vi "ActiveObjects_DynamicEvents.vi"(7 "Action":T2=enum."GeneratePattern", 8 "error in (no error)":errorcluster, 10 "DataIn":variant, 11 "ClassRefToActOn":refnum<vi>) -> (0 "error out":errorcluster, 1 "Name":string, 2 "DataOut":variant, 3 "Cancelled":bool)   [LabVIEW 2020]
uses:
  Provider_BaseClassInterface/BaseProvider_SubVIs/BaseProvider_DesignPatternsActions.ctl
  Common/LvClass_class/GDSLvClass_ProviderTypes.ctl
  Provider_EndevoGOOP400/EndevoG4ProviderName.ctl
  Common/CommonVIs/CommonVIs_AttributeDataType.ctl
  <vilib>/picture/picture.llb/imagedata.ctl
  Common/LvIcon_class/subvis/GDSLvIcon_TextDataType.ctl
  Common/LvIcon_class/GDSLvIcon_WordCompressionType.ctl
  Common/LvIcon_class/GDSLvIcon_TextAlignment.ctl
  <vilib>/Utility/lvfile.llb/NI_FileType.lvlib
panel:
  out "NameExist4":string
  in  "AddWindowControlVI":bool
  in  "WindowControlName":string caption="Enter process window control VI name"
  in  "ProcessCreation":T1(ring) caption="Process creation"
  out "NameExist1":string
  out "NameExist3":string
  out "NameExist2":string
  in  "AddInDestructor":bool
  in  "AddInConstructor":bool
  in  "StopName":string caption="Enter Stop Process Name"
  in  "StartName":string caption="Enter Start Process Name"
  in  "_Cancel":bool
  in  "_OK":bool
  in  "ProcessName":string caption="Enter Active Process Name"
  # "Active Object using Dymanic Events"
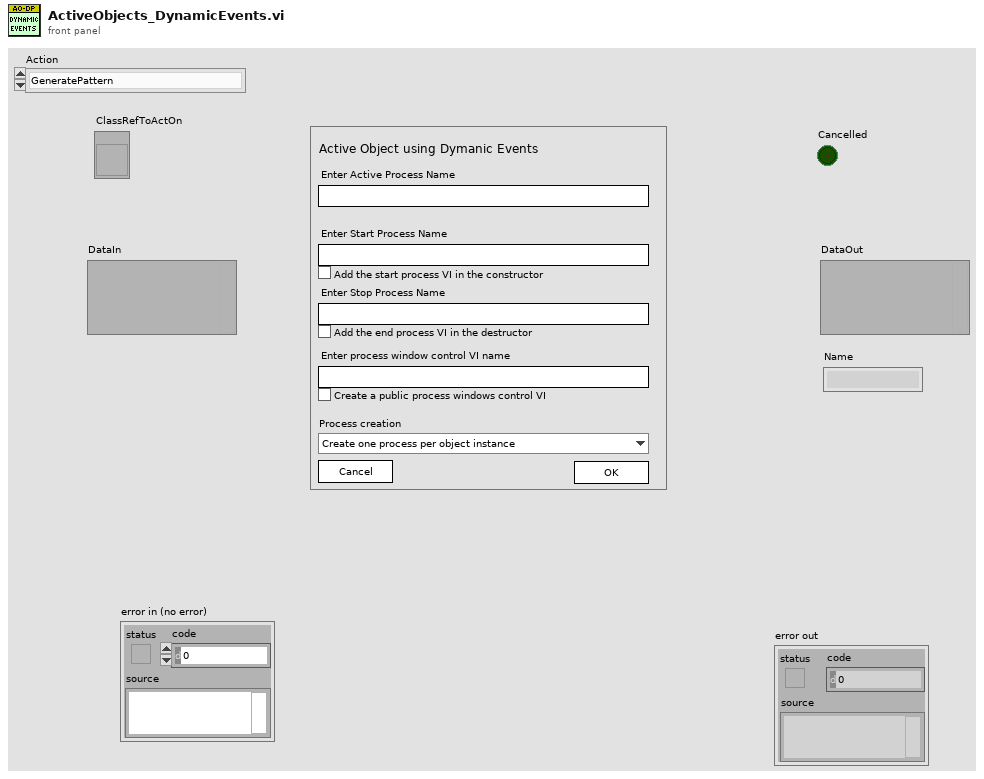
[diagram p1: front panel]
types:
  T1 = enum16{"Create one process per object instance", "Create only one process for this class"}
  T2 = typedef "BaseProvider_DesignPatternsActions.ctl" = enum16{"AddPatternDialog", "GeneratePattern", "RemovePattern", "CreatePatternMethod", "UpdatePattern"}
  T3 = typedef "GDSLvClass_ProviderTypes.ctl" = enum16{"UnKnown(LabVOOP)", "Native", "EndevoGOOP3", "OpenG(RootObject)", "OpenG(OpenG_Object)", "EndevoGOOP4", "JKI1"}
  T4 = cluster{"Data":cluster{"ProcessName":string, "StartName":string, "StopName":string, "AddInConstructor":bool, "AddInDestructor":bool, "ProcessCreation":enum16{"Create one process per object instance", "Create only one process for this class"}, "WindowControlName":string, "AddWindowControlVI":bool}, "ClassFolder":path, "SupportFolder":path, "ProcessCtl":refnum<vi>, "ProtectedFolder":refnum<vi>, "ProcessVI":refnum<vi>, "StartVI":refnum<vi>, "StopVI":refnum<vi>, "Application":refnum<vi>, "RepositoryVI":refnum<vi>, "ProcessIdRef":refnum<vi>, "ProcessRepository":path, "ClassProvider":T3, "TemplateName":string, "VI_ToFind":path, "MethodTemplate":path, "VI":refnum<vi>, "VI_ToFindSingleton":path, "Name":string, "WindowControlVI":refnum<vi>, "ClassType":enum16{"4x4x4", "5x6x5", "6x8x6", "4x4x4_Singleton", "5x6x5_Singleton", "6x8x6_Singleton"}}
  T5 = cluster{"ProcessName":string, "StartName":string, "StopName":string, "AddInConstructor":bool, "AddInDestructor":bool, "ProcessCreation":enum16{"Create one process per object instance", "Create only one process for this class"}, "WindowControlName":string, "AddWindowControlVI":bool}
  T6 = enum8{"Enabled", "Disabled", "Disabled and Grayed Out"}
  T7 = cluster{"Cancelled":bool, "Files":path[], "ClassPath":path, "DataOut":variant, "Name":string}
  T8 = typedef "EndevoG4ProviderName.ctl" = enum16{"EndevoGOOP400"}
  T9 = enum16{"4x4x4", "5x6x5", "6x8x6", "4x4x4_Singleton", "5x6x5_Singleton", "6x8x6_Singleton"}
  T10 = enum32{"invalid VI type", "Standard VI", "Control VI", "Global VI", "Polymorphic VI", "Configuration VI", "SubSystem", "Facade VI", "Method VI"}
  T11 = typedef "GDSLvIcon_TextDataType.ctl" = cluster{"Text":string, "Allow Only Capital Chars":bool, "Compression":T12, "Alignment":T13}
  T12 = typedef "GDSLvIcon_WordCompressionType.ctl" = enum16{"Auto", "On", "Off"}
  T13 = typedef "GDSLvIcon_TextAlignment.ctl" = enum16{"Center", "Left", "Right"}
  T14 = typedef "imagedata.ctl" = cluster{"image type":i32, "image depth":i32, "image":u8[], "mask":u8[], "colors":u32[], "Rectangle":cluster{"left":i16, "top":i16, "right":i16, "bottom":i16}}
  T15 = typedef "GDSLvCLass_ClassSettingsType.ctl" = cluster{"ClassProviderName":string, "ClassTemplateUsed":string, "ClassTemplateVersion":string, "ClassDescription":string, "PlugIns":T16[], "ConnectorPanePattern":string}
  T16 = typedef "GDSLvClass_PlugIn.ctl" = cluster{"Type":T17, "ID":string, "Version":string, "Path":path, "Name":string, "Data":variant}
  T17 = typedef "GDSLvClass_PlugInTypes.ctl" = enum16{"DesignPattern", "MethodTypes"}
  T18 = typedef "GOOP400_Options.ctl" = cluster{"FlatFolderStructure":bool}
  T19 = enum32{"invalid scope", "public", "private", "protected"}[]
  T20 = typedef "CommonVIs_AttributeDataType.ctl" = enum16{"UINT8", "INT8", "UINT16", "INT16", "UINT32", "INT32", "UINT64", "INT64", "SGL", "DBL", "EXT", "CSG", "CDB", "CXT", "TimeStamp", "STRING", "PATH", "BOOL", "ENUM", "RefNum", "VIRefNum", "LabVIEW Class", "Cluster", "Variant", "TypeDef", "Waveform", "LabVIEW Object", "Other", "void", "Set", "Map"}
  T21 = typedef "GDSLvClass_IconSettingsType.ctl" = cluster{"Frame":u32, "Frame thickness":u8, "Header Background":u32, "Header Text":u32, "ColorPublic":u32, "ColorProtected":u32, "ColorPrivate":u32, "Body Text":u32, "ClassBodyIcon":string}
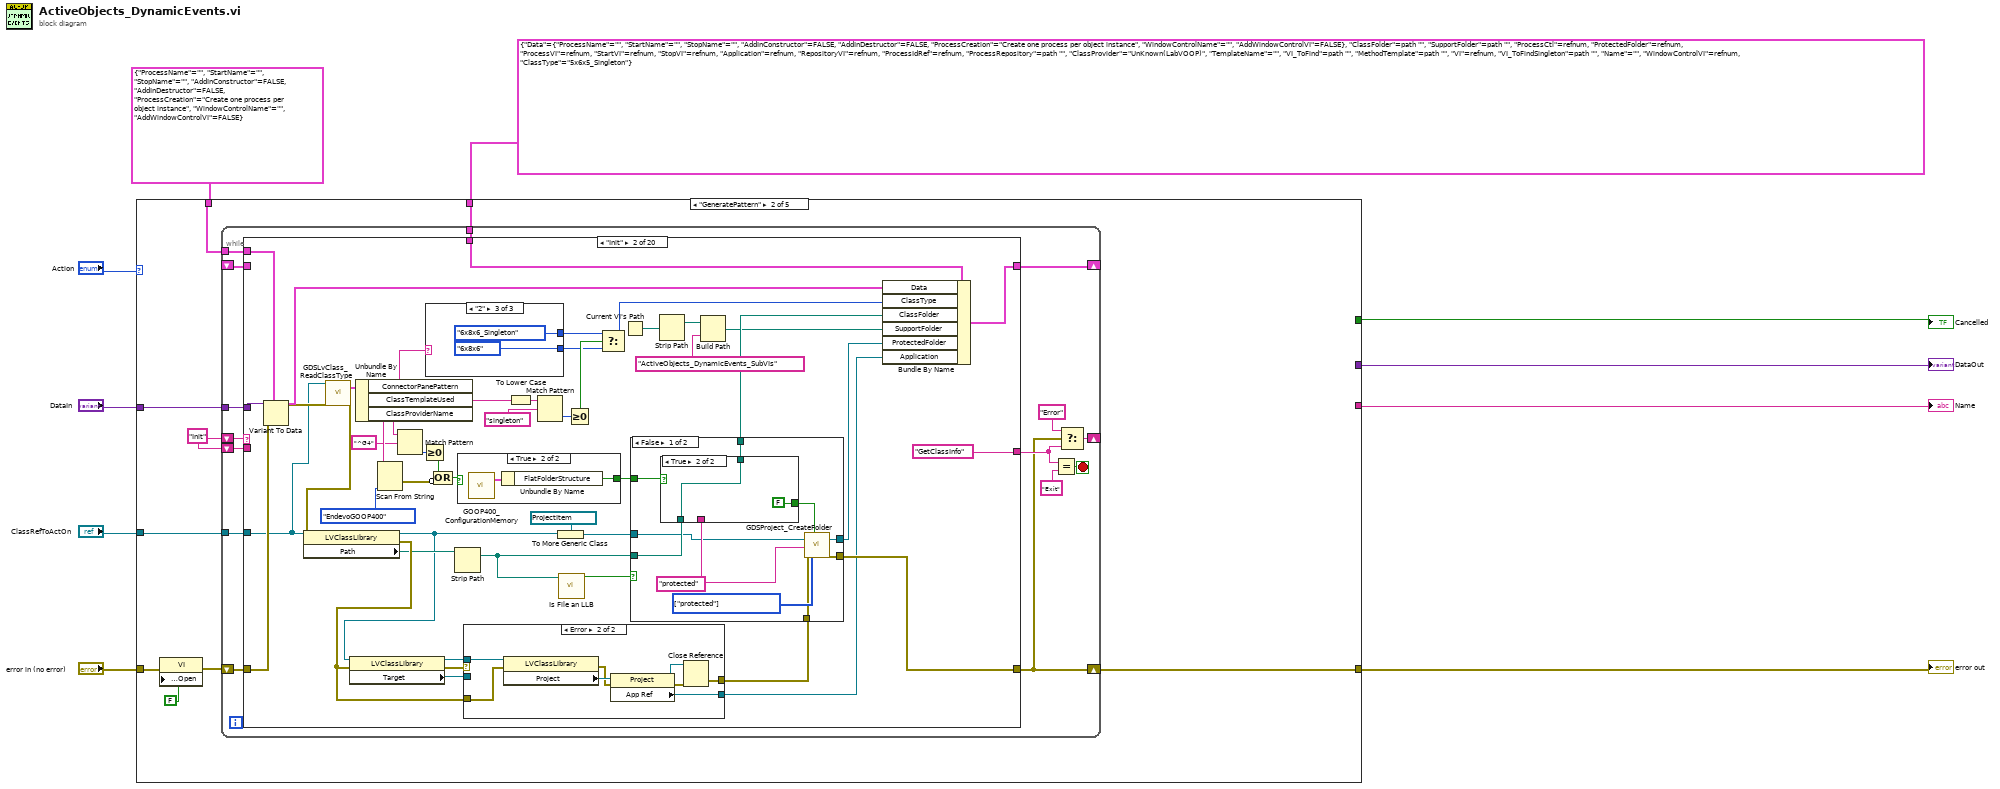
[diagram p0: block diagram]
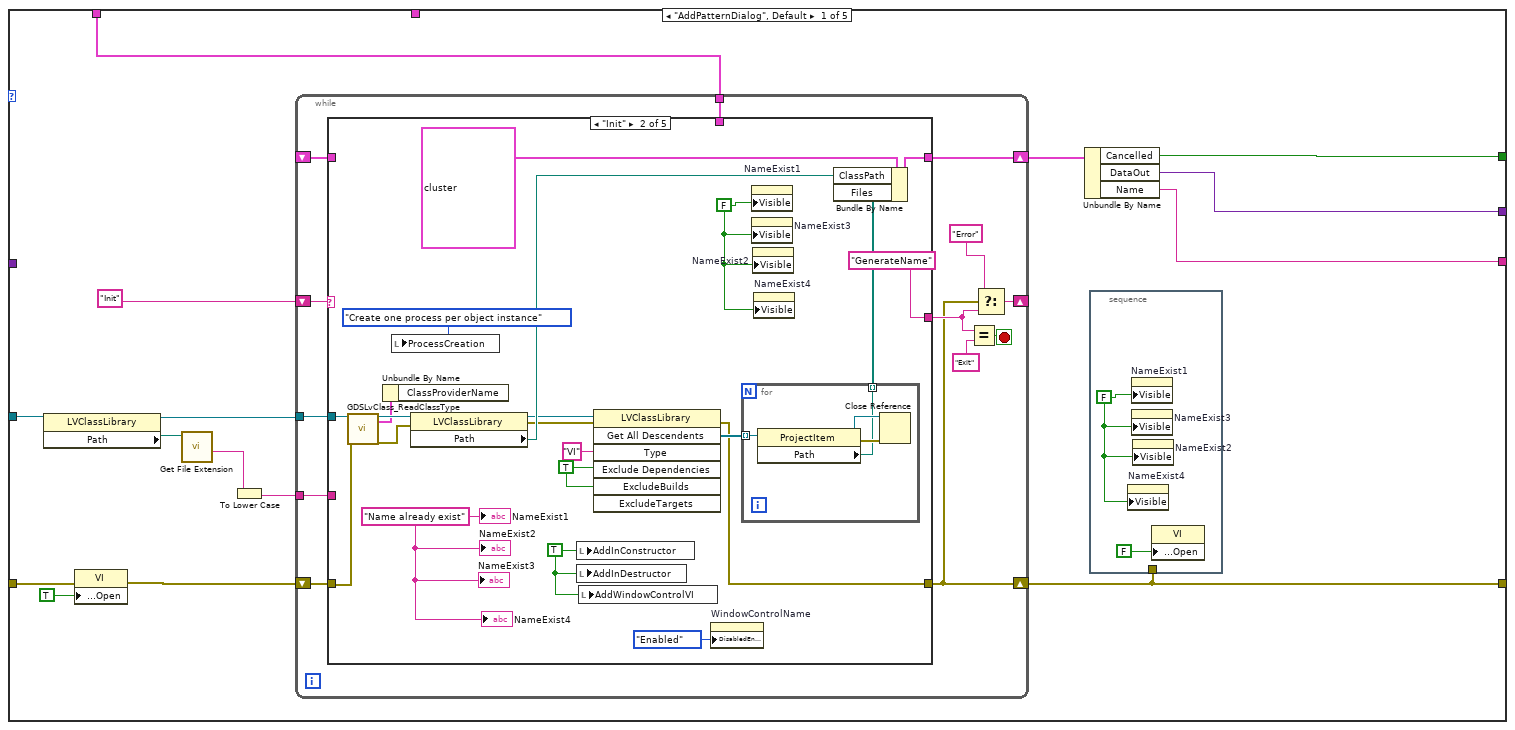
[diagram p2: hidden frame]
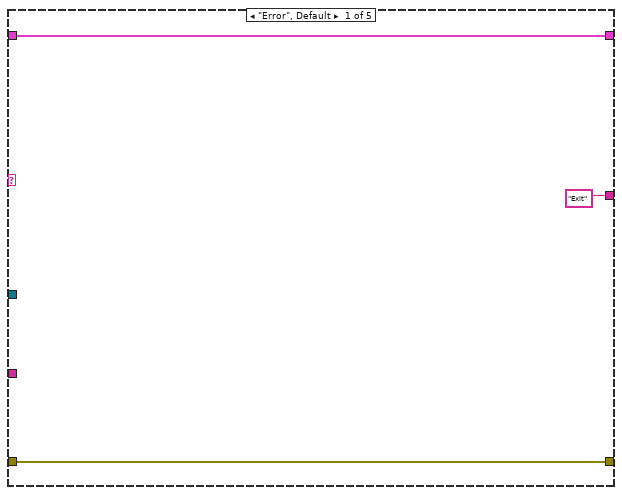
[diagram p3: hidden frame]
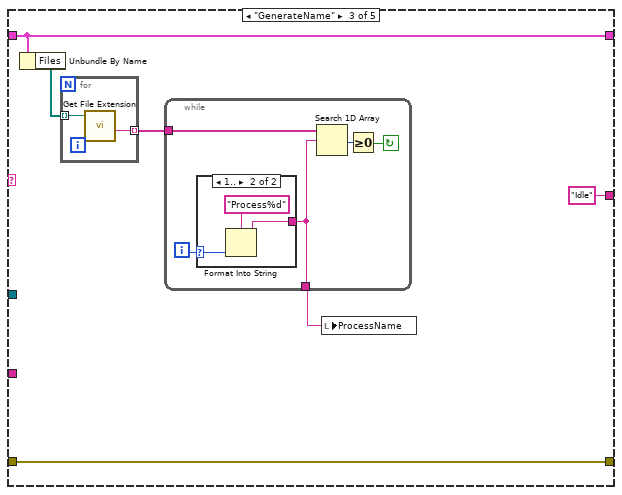
[diagram p4: hidden frame]
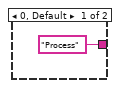
[diagram p5: hidden frame]
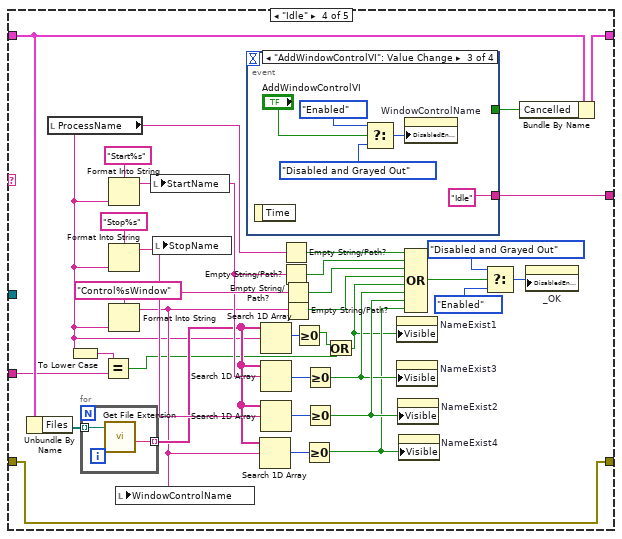
[diagram p6: hidden frame]
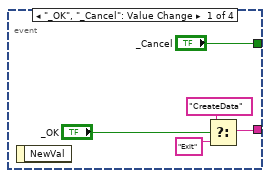
[diagram p7: hidden frame]
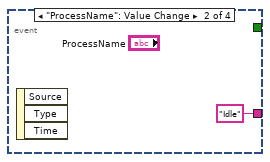
[diagram p8: hidden frame]
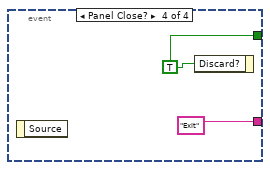
[diagram p9: hidden frame]
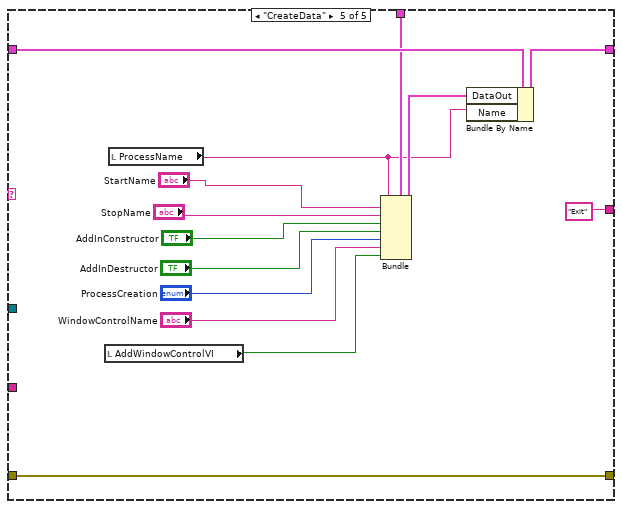
[diagram p10: hidden frame]
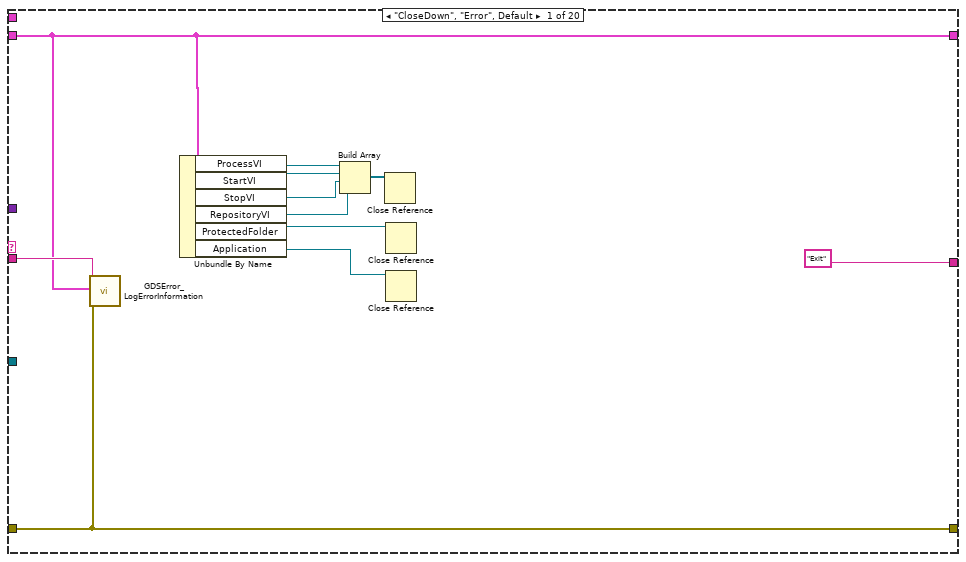
[diagram p11: hidden frame]
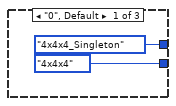
[diagram p13: hidden frame]
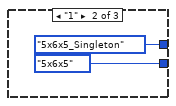
[diagram p14: hidden frame]
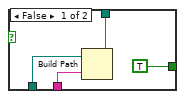
[diagram p15: hidden frame]
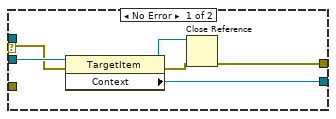
[diagram p17: hidden frame]
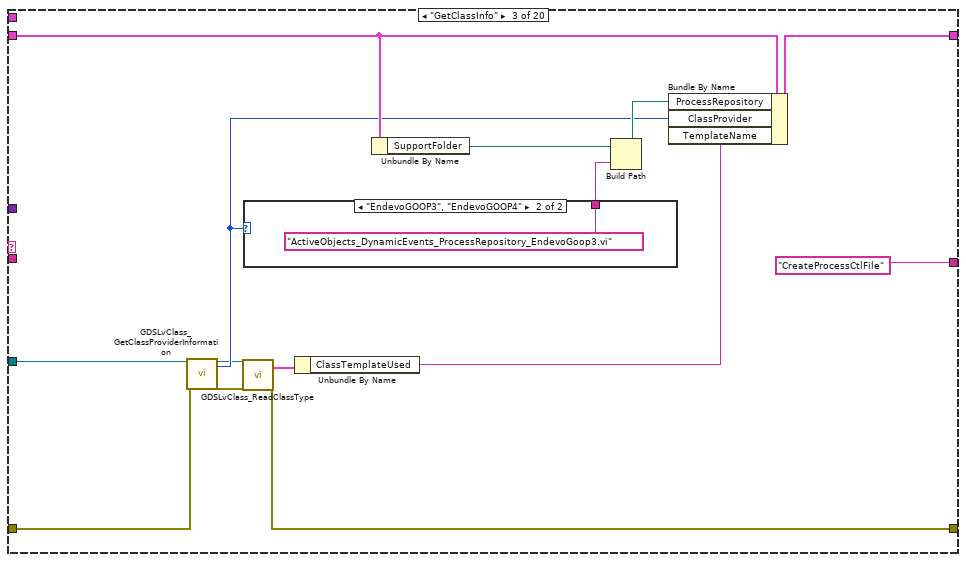
[diagram p18: hidden frame]
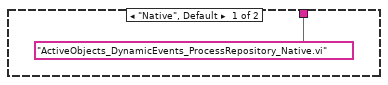
[diagram p19: hidden frame]
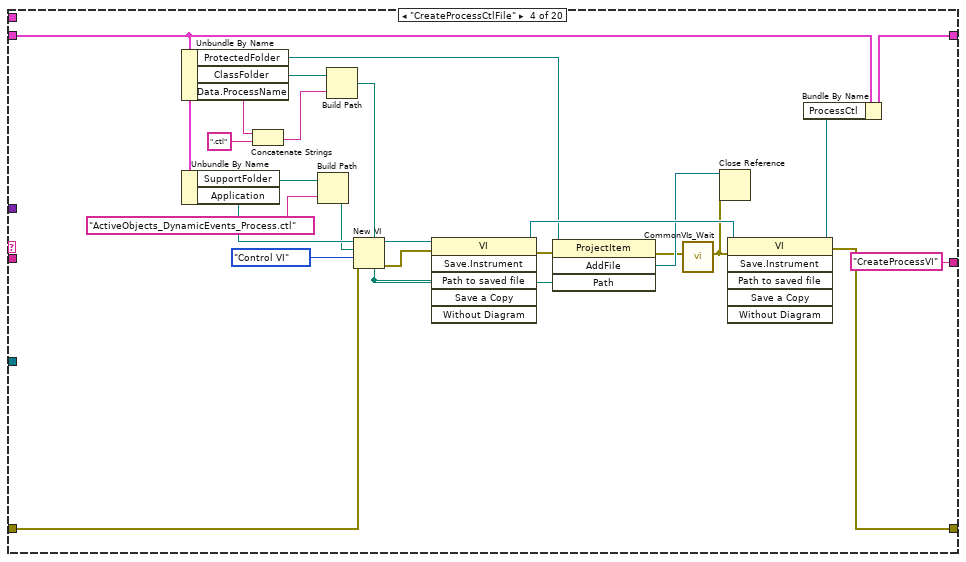
[diagram p20: hidden frame]
diagram:
  n1 = case shown="\"GeneratePattern\"" "Action" {
    tunnel: "error in (no error)" -> [w24 w151 w883 w884 w890]
    tunnel: [w21 w157 w883 w884 w885] -> w8
    tunnel: "ClassRefToActOn" -> [w15 w153 _ _ w889]
    tunnel: [w19 _ _ _ _] -> w6
    tunnel: [w18 _ _ _ _] -> w5
    tunnel: T5 {"ProcessName"="", "StartName"="", "StopName"="", "AddInConstructor"=FALSE, "AddInDestructor"=FALSE, "ProcessCreation"=enum."Create one process per object instance", "WindowControlName"="", "AddWindowControlVI"=FALSE} ("output cluster") -> [w17 w155 _ _ w886]
    tunnel: "DataIn" -> [_ w156 _ _ w888]
    tunnel: T4 {"Data"={"ProcessName"="", "StartName"="", "StopName"="", "AddInConstructor"=FALSE, "AddInDestructor"=FALSE, "ProcessCreation"=enum."Create one process per object instance", "WindowControlName"="", "AddWindowControlVI"=FALSE}, "ClassFolder"=path "", "SupportFolder"=path "", "ProcessCtl"=refnum, "ProtectedFolder"=refnum, "ProcessVI"=refnum, "StartVI"=refnum, "StopVI"=refnum, "Application"=refnum, "RepositoryVI"=refnum, "ProcessIdRef"=refnum, "ProcessRepository"=path "", "ClassProvider"=enum."UnKnown(LabVOOP)", "TemplateName"="", "VI_ToFind"=path "", "MethodTemplate"=path "", "VI"=refnum, "VI_ToFindSingleton"=path "", "Name"="", "WindowControlVI"=refnum, "ClassType"=enum."5x6x5_Singleton"} -> [_ w154 _ _ w887]
    tunnel: [w16 _ _ _ _] -> w1
    frame "AddPatternDialog", Default {
      n2 = property class="LVClassLibrary"(reference=w15) -> (reference out=w14:refnum<vi>, "Path"=w13:path)  [unwired: 1 in, 1 out]
      n3 = property class="VI"(error in=w24, "Front Panel.Open"=TRUE ("Front Panel Window:Open")) -> (error out=w23:errorcluster)  [unwired: 1 in, 1 out]
      n4 = call <vilib>:"Get File Extension.vi"("file"=w13) -> ("filename without extension"=w11:string)  [unwired: 6 in, 4 out]
      n5 = To Lower Case(string=w11) -> (all lower case string=w12:string)
      n6 = while {
        shift-right: [w33] -> w21
        shift-left: w23 -> [w40]
        shift-right: [w38] -> _
        shift-left: "Init" -> [w39]
        shift-right: [w32] -> w20
        shift-left: _ -> [w31]
        tunnel: w14 -> [w30]
        tunnel: w17 -> [w29]
        tunnel: w12 -> [w28]
        stop <- w37 stop-if-true
        n7 = case shown="\"Init\"" w39 {
          tunnel: w40 -> [w43 w51 w69 w103 w142]
          tunnel: [w43 w60 w69 w103 w142] -> w33
          tunnel: ["Exit" "GenerateName" "Idle" w119 "Exit"] -> w34
          tunnel: [w41 w58 w70 w118 w144] -> w32
          tunnel: w31 -> [w41 _ w70 w113 w146]
          tunnel: w30 -> [_ w53 _ _ _]
          tunnel: w29 -> [_ _ _ _ w141]
          tunnel: w28 -> [_ _ _ w87 _]
          frame "Error", Default {
          }
          frame "Init" {
            w46 = "Name already exist" ("NameExist1")
            w45 = FALSE ("Visible")
            w47 = TRUE ("AddInConstructor")
            w62 = TRUE ("ExcludeDependencies")
            n8 = call "GDSLvClass_ReadClassType.vi"("Class Refnum In"=w53, "error in (no error)"=w51) -> ("Class Refnum Out"=w52:refnum<vi>, "ClassSettings"=w49:T15, "error out"=w50:errorcluster)  [unwired: 15 in]
            n9 = Unbundle By Name(w49) -> ()  [unwired: 1 out]
            n10 = local write "ProcessCreation"(T1."Create one process per object instance" ("ProcessCreation")) -> ()
            n11 = property class="LVClassLibrary"(reference=w52, error in=w50) -> (reference out=w55:refnum<vi>, error out=w54:errorcluster, "Path"=w57:path)
            n12 = local write "AddInConstructor"(w47) -> ()
            n13 = local write "AddInDestructor"(w47) -> ()
            n14 = local write "AddWindowControlVI"(w47) -> ()
            n15 = invoke class="LVClassLibrary" method="Get All Descendents"(reference=w55, error in=w54, "Type"="VI", "Exclude Dependencies"=w62, "ExcludeBuilds"=w62) -> (error out=w60:errorcluster, "All Descendents"=w61:refnum<vi>[])  [unwired: 2 in, 5 out]
            n16 = property on="WindowControlName" class="Str"("DisabledEnum"=T6."Enabled" ("Disabled")) -> ()  [unwired: 2 in, 2 out]
            n17 = for {
              tunnel: w61 -> [w68] mode=indexing
              tunnel: [w65] -> w56 mode=indexing
              n18 = property class="ProjectItem"(reference=w68) -> (reference out=w66:refnum<vi>, error out=w67:errorcluster, "Path"=w65:path)  [unwired: 1 in]
              n19 = Close Reference(reference=w66, error in (no error)=w67) -> ()  [unwired: 1 out]
            }
            n20 = property on="NameExist1" class="Str"("Visible"=w45) -> ()  [unwired: 2 in, 2 out]
            n21 = property on="NameExist3" class="Str"("Visible"=w45) -> ()  [unwired: 2 in, 2 out]
            n22 = property on="NameExist2" class="Str"("Visible"=w45) -> ()  [unwired: 2 in, 2 out]
            n23 = property on="NameExist4" class="Str"("Visible"=w45) -> ()  [unwired: 2 in, 2 out]
            n24 = Bundle By Name(cluster=T7 {"Cancelled"=FALSE, "Files"=[], "ClassPath"=path "", "DataOut"=variant, "Name"=""}, "ClassPath"=w57, "Files"=w56) -> (w58:T7)
            "NameExist2" <- w46
            "NameExist3" <- w46
            "NameExist1" <- w46
            "NameExist4" <- w46
          }
          frame "GenerateName" {
            n25 = Unbundle By Name(w70) -> ("Files"=w74:path[])
            n26 = for {
              tunnel: w74 -> [w85] mode=indexing
              tunnel: [w84] -> w73 mode=indexing
              n27 = call <vilib>:"Get File Extension.vi"("file"=w85) -> ("filename without extension"=w84:string)  [unwired: 6 in, 4 out]
            }
            n28 = while {
              tunnel: w73 -> [w78]
              tunnel: [w75] -> w72
              i -> [w79]
              stop <- w76 continue-if-true
              n29 = case shown="1.." w79 {
                selector: w79 -> [_ w82]
                tunnel: ["Process" ("format string") w81] -> w75
                frame 0, Default {
                }
                frame 1.. {
                  n30 = Format Into String(format string="Process%d", w82) -> (resulting string=w81:string)  [unwired: 2 in, 1 out]
                }
              }
              n31 = Search 1D Array(1D array=w78, element=w75) -> (index of element=w77:i32)  [unwired: 1 in]
              n32 = Greater Or Equal To 0?(x=w77) -> (x >= 0?=w76:bool)
            }
            n33 = local write "ProcessName"(w72) -> ()
          }
          frame "Idle" {
            n34 = Unbundle By Name(w113) -> ("Files"=w114:path[])
            n35 = local read "ProcessName"() -> (w89:string)
            n36 = To Lower Case(string=w89) -> (all lower case string=w88:string)
            n37 = for {
              tunnel: w114 -> [w121] mode=indexing
              tunnel: [w120] -> w100 mode=indexing
              n38 = call <vilib>:"Get File Extension.vi"("file"=w121) -> ("filename without extension"=w120:string)  [unwired: 6 in, 4 out]
            }
            n39 = Equal?(x=w88, y=w87) -> (x = y?=w86:bool)
            n40 = Format Into String(format string="Start%s", w89) -> (resulting string=w107:string)  [unwired: 2 in, 1 out]
            n41 = Format Into String(format string="Stop%s", w89) -> (resulting string=w108:string)  [unwired: 2 in, 1 out]
            n42 = Format Into String(format string="Control%sWindow", w89) -> (resulting string=w98:string)  [unwired: 2 in, 1 out]
            n43 = local write "WindowControlName"(w98) -> ()
            n44 = local write "StartName"(w107) -> ()
            n45 = local write "StopName"(w108) -> ()
            n46 = event shown="[2] \"AddWindowControlVI\": Value Change" {
              selector: _ -> [_ _ _ _]
              dyn-events: _ -> [_ _ _ _]
              timeout: _ -> [_ _ _ _]
              tunnel: [w125 "Idle" "Idle" "Exit"] -> w119
              tunnel: ["_Cancel" _ _ w133] -> w117
              event "_OK", "_Cancel": Value Change {
                n47 = event-data() -> ()  [unwired: 1 in, 1 out]
                n48 = Select(t="CreateData", s="_OK", f="Exit") -> (s? t:f=w125:string)
              }
              event "ProcessName": Value Change {
                n49 = event-data() -> ()  [unwired: 1 in, 3 out]
              }
              event "AddWindowControlVI": Value Change {
                n50 = event-data() -> ()  [unwired: 1 in, 1 out]
                n51 = Select(t=T6."Enabled" ("Disabled"), s="AddWindowControlVI", f=T6."Disabled and Grayed Out" ("Disabled")) -> (s? t:f=w130:T6)
                n52 = property on="WindowControlName" class="Str"("DisabledEnum"=w130) -> ()  [unwired: 2 in, 2 out]
              }
              event Panel Close? {
                w133 = TRUE ("Discard?")
                n53 = event-data() -> ()  [unwired: 1 in, 1 out]
                n54 = event-data("Discard?"=w133) -> ()  [unwired: 1 in, 1 out]
              }
            }
            n55 = Search 1D Array(1D array=w100, element=w98) -> (index of element=w101:i32)  [unwired: 1 in]
            n56 = Search 1D Array(1D array=w100, element=w89) -> (index of element=w112:i32)  [unwired: 1 in]
            n57 = Search 1D Array(1D array=w100, element=w107) -> (index of element=w111:i32)  [unwired: 1 in]
            n58 = Search 1D Array(1D array=w100, element=w108) -> (index of element=w110:i32)  [unwired: 1 in]
            n59 = Empty String/Path?(string/path=w89) -> (empty?=w104:bool)
            n60 = Empty String/Path?(string/path=w107) -> (empty?=w105:bool)
            n61 = Empty String/Path?(string/path=w108) -> (empty?=w106:bool)
            n62 = Empty String/Path?(string/path=w98) -> (empty?=w97:bool)
            n63 = Greater Or Equal To 0?(x=w112) -> (x >= 0?=w91:bool)
            n64 = Greater Or Equal To 0?(x=w101) -> (x >= 0?=w96:bool)
            n65 = Greater Or Equal To 0?(x=w111) -> (x >= 0?=w102:bool)
            n66 = Greater Or Equal To 0?(x=w110) -> (x >= 0?=w109:bool)
            n67 = Or(x=w91, y=w86) -> (x .or. y?=w90:bool)
            n68 = property on="NameExist1" class="Str"("Visible"=w90) -> ()  [unwired: 2 in, 2 out]
            n69 = property on="NameExist3" class="Str"("Visible"=w102) -> ()  [unwired: 2 in, 2 out]
            n70 = property on="NameExist2" class="Str"("Visible"=w109) -> ()  [unwired: 2 in, 2 out]
            n71 = property on="NameExist4" class="Str"("Visible"=w96) -> ()  [unwired: 2 in, 2 out]
            n72 = Compound Arithmetic op=OR(w104, w105, w106, w97, w90, w102, w109, w96) -> (w95:bool)
            n73 = Select(t=T6."Disabled and Grayed Out" ("Disabled"), s=w95, f=T6."Enabled" ("Disabled")) -> (s? t:f=w94:T6)
            n74 = Bundle By Name(cluster=w113, "Cancelled"=w117) -> (w118:T7)
            n75 = property on="_OK" class="Bool"("DisabledEnum"=w94) -> ()  [unwired: 2 in, 2 out]
          }
          frame "CreateData" {
            n76 = local read "AddWindowControlVI"() -> (w135:bool)
            n77 = local read "ProcessName"() -> (w139:string)
            n78 = Bundle(cluster=w141, "ProcessName"=w139, "StartName"="StartName", "StopName"="StopName", "AddInConstructor"="AddInConstructor", "AddInDestructor"="AddInDestructor", "ProcessCreation"="ProcessCreation", "WindowControlName"="WindowControlName", "AddWindowControlVI"=w135) -> (w145:T5)
            n79 = Bundle By Name(cluster=w146, "DataOut"=w145, "Name"=w139) -> (w144:T7)
          }
        }
        n80 = Equal?(x=w34, y="Exit") -> (x = y?=w37:bool)
        n81 = Select(t="Error", s=w33, f=w34) -> (s? t:f=w38:string)
      }
      n82 = Unbundle By Name(w20) -> ("Cancelled"=w19:bool, "DataOut"=w18:variant, "Name"=w16:string)
      n83 = stacked-sequence {
        tunnel: w21 -> [_]
        frame #0 {
          w26 = FALSE ("Visible")
          n84 = property on="NameExist4" class="Str"("Visible"=w26) -> ()  [unwired: 2 in, 2 out]
          n85 = property on="NameExist1" class="Str"("Visible"=w26) -> ()  [unwired: 2 in, 2 out]
          n86 = property on="NameExist3" class="Str"("Visible"=w26) -> ()  [unwired: 2 in, 2 out]
          n87 = property on="NameExist2" class="Str"("Visible"=w26) -> ()  [unwired: 2 in, 2 out]
          n88 = property class="VI"("Front Panel.Open"=FALSE ("Front Panel Window:Open")) -> ()  [unwired: 2 in, 2 out]
        }
      }
    }
    frame "GeneratePattern" {
      w149 = "Init"
      n89 = property class="VI"(error in=w151, "Front Panel.Open"=FALSE ("Front Panel Window:Open")) -> (error out=w150:errorcluster)  [unwired: 1 in, 1 out]
      n90 = while {
        shift-right: [w165] -> w157
        shift-left: w150 -> [w172]
        shift-right: [w170] -> _
        shift-left: w149 -> [w171]
        shift-right: [w164] -> _
        shift-left: _ -> [w163]
        tunnel: w156 -> [w162]
        tunnel: w155 -> [w161]
        tunnel: w154 -> [w160]
        tunnel: w153 -> [w159]
        shift-left: w149 -> [w158]
        stop <- w169 stop-if-true
        n91 = case shown="\"Init\"" w171 {
          tunnel: w172 -> [w175 w224 w283 w307 w331 w356 w383 w412 w444 w460 w471 w511 w529 w595 w609 w630 w687 w757 w810 w869]
          tunnel: [w175 w218 w274 w294 w318 w344 w372 w399 w435 w450 w468 w494 w539 w586 w608 w631 w686 w755 w808 w876] -> w165
          tunnel: ["Exit" "GetClassInfo" "CreateProcessCtlFile" "CreateProcessVI" "CreateStartProcessVI" "CreateStopProcessVI" w365 "CreateProcessRepositoryVI" w428 "UpdateOORefInVIs" w467 "UpdateVIs" "UpdateRepositoryStaticVI" w597 "FixViRefType" "UpdateIcons" "UpdateCreate?" "UpdateDestroy?" "SaveAll" "CloseDown"] -> w166
          tunnel: [w178 w229 w277 w297 w321 w347 w374 w401 w437 w454 w475 w509 w533 w580 w605 w665 w689 w753 w806 w873] -> w164
          tunnel: w163 -> [w178 _ w280 w298 w322 w338 w367 w402 w426 w455 w475 w509 w533 w580 w605 w665 w689 w753 w806 w873]
          tunnel: w162 -> [_ w228 _ _ _ _ _ _ _ _ _ _ _ _ _ _ _ _ _ _]
          tunnel: w161 -> [_ w227 _ _ _ _ _ _ _ _ _ _ _ _ _ _ _ _ _ _]
          tunnel: w160 -> [_ w226 _ _ _ _ _ _ _ _ _ _ _ _ _ _ _ _ _ _]
          tunnel: w159 -> [_ w205 w284 _ _ _ _ w393 _ w452 w470 w500 _ _ w606 _ w693 w752 w805 w875]
          tunnel: w158 -> [w182 _ _ _ _ _ _ _ _ _ _ _ _ _ _ _ _ _ _ _]
          frame "CloseDown", "Error", Default {
            n92 = call "GDSError_LogErrorInformation.vi"("State"=w182, "LocalVariableData"=w178, "error in (no error)"=w175) -> ()  [unwired: 16 in, 1 out]
            n93 = Unbundle By Name(w178) -> ("ProcessVI"=w181:refnum<vi>, "StartVI"=w180:refnum<vi>, "StopVI"=w179:refnum<vi>, "RepositoryVI"=w177:refnum<vi>, "ProtectedFolder"=w174:refnum<vi>, "Application"=w173:refnum<vi>)
            n94 = Build Array(w181, w180, w179, w177) -> (w176:refnum<vi>[])
            n95 = Close Reference(reference=w176) -> ()  [unwired: 1 in, 1 out]
            n96 = Close Reference(reference=w174) -> ()  [unwired: 1 in, 1 out]
            n97 = Close Reference(reference=w173) -> ()  [unwired: 1 in, 1 out]
          }
          frame "Init" {
            n98 = Variant To Data(error in=w224, type=w227, Variant=w228) -> (data=w225:T5, error out=w207:errorcluster)
            n99 = call "GDSLvClass_ReadClassType.vi"("Class Refnum In"=w205, "error in (no error)"=w207) -> ("ClassSettings"=w200:T15, "error out"=w206:errorcluster)  [unwired: 15 in, 1 out]
            n100 = property class="LVClassLibrary"(reference=w205, error in=w206) -> (reference out=w194:refnum<vi>, error out=w213:errorcluster, "Path"=w210:path)
            n101 = property class="LVClassLibrary"(reference=w194, error in=w213) -> (reference out=w216:refnum<vi>, error out=w214:errorcluster, "Target"=w215:refnum<vi>)
            n102 = Unbundle By Name(w200) -> ("ConnectorPanePattern"=w204:string, "ClassTemplateUsed"=w189:string, "ClassProviderName"=w192:string)
            n103 = Scan From String(input string=w192, default 1=EndevoG4ProviderName."EndevoGOOP400" ("ProviderName")) -> (error out=w186:errorcluster)  [unwired: 4 in, 2 out]
            n104 = Match Pattern(string=w189, regular expression="^G4") -> (offset past match=w187:i32)  [unwired: 1 in, 3 out]
            n105 = Greater Or Equal To 0?(x=w187) -> (x >= 0?=w185:bool)
            n106 = case shown="\"2\"" w204 {
              tunnel: [T9."4x4x4" ("ClassType") T9."5x6x5" ("ClassType") T9."6x8x6" ("ClassType")] -> w198
              tunnel: [T9."4x4x4_Singleton" ("ClassType") T9."5x6x5_Singleton" ("ClassType") T9."6x8x6_Singleton" ("ClassType")] -> w197
              frame "0", Default {
              }
              frame "1" {
              }
              frame "2" {
              }
            }
            n107 = Compound Arithmetic op=OR(w185, invert w186) -> (w184:bool)
            n108 = Strip Path(path=w210) -> (stripped path=w208:path)  [unwired: 1 out]
            n109 = case shown="True" w184 {
              tunnel: [_ w231] -> w190
              frame False {
              }
              frame True {
                n110 = call "GOOP400_ConfigurationMemory.vi"() -> ("OptionsOut"=w232:T18)  [unwired: 18 in, 1 out]
                n111 = Unbundle By Name(w232) -> ("FlatFolderStructure"=w231:bool)
              }
            }
            n112 = case shown="Error" w214 {
              selector: w214 -> [w259 _]
              tunnel: w215 -> [w263 _]
              tunnel: [w262 w265] -> w212
              tunnel: [w258 w266] -> w211
              tunnel: w216 -> [_ w271]
              tunnel: w213 -> [_ w270]
              frame No Error {
                n113 = property class="TargetItem"(reference=w263, error in=w259) -> (reference out=w260:refnum<vi>, error out=w261:errorcluster, "Context"=w262:refnum<vi>)
                n114 = Close Reference(reference=w260, error in (no error)=w261) -> (error out=w258:errorcluster)
              }
              frame Error {
                n115 = property class="LVClassLibrary"(reference=w271, error in=w270) -> (error out=w264:errorcluster, "Project"=w269:refnum<vi>)  [unwired: 1 out]
                n116 = property class="Project"(reference=w269, error in=w264) -> (reference out=w267:refnum<vi>, error out=w268:errorcluster, "App Ref"=w265:refnum<vi>)
                n117 = Close Reference(reference=w267, error in (no error)=w268) -> (error out=w266:errorcluster)
              }
            }
            n118 = To Lower Case(string=w189) -> (all lower case string=w202:string)
            n119 = Match Pattern(string=w202, regular expression="singleton" ("search string")) -> (offset past match=w203:i32)  [unwired: 1 in, 3 out]
            n120 = To More Generic Class(target class=refnum<vi> refnum ("AddItem"), reference=w194) -> (generic class reference=w193:refnum<vi>)
            n121 = call <vilib>:"Is File an LLB.vi"("path"=w208) -> ("Is LLB?"=w209:bool)  [unwired: 9 in, 1 out]
            n122 = Greater Or Equal To 0?(x=w203) -> (x >= 0?=w199:bool)
            n123 = Select(t=w197, s=w199, f=w198) -> (s? t:f=w196:T9)
            n124 = Current VI's Path() -> (path=w222:path)
            n125 = case shown="False" w209 {
              tunnel: [w245 w256] -> w223
              tunnel: [w244 w257] -> w218
              tunnel: [w243 w255] -> w217
              tunnel: w193 -> [w240 w255]
              tunnel: w211 -> [w242 w257]
              tunnel: w208 -> [w241 w256]
              tunnel: w190 -> [w239 _]
              frame False {
                w248 = T19 [enum."protected"] items=["invalid scope", "public", "private", "protected"] ("FolderScope")
                w247 = "protected" ("name or relative path")
                n126 = case shown="True" w239 {
                  tunnel: w247 -> [w252 _]
                  tunnel: [TRUE ("CreateThePhysicalFolderIfPossible(False)") FALSE ("CreateThePhysicalFolderIfPossible(False)")] -> w246
                  tunnel: [w250 w253] -> w245
                  tunnel: w241 -> [w249 w253]
                  frame False {
                    n127 = Build Path(base path=w249, name or relative path=w252) -> (appended path=w250:path)
                  }
                  frame True {
                  }
                }
                n128 = call "GDSProject_CreateFolder.vi"("Project Item To Create Folder Below(Use MyComputer if not wired)"=w240, "FolderName"=w247, "error in (no error)"=w242, "FolderScope"=w248, "CreateThePhysicalFolderIfPossible(False)"=w246) -> ("ItemOut"=w243:refnum<vi>, "error out"=w244:errorcluster)  [unwired: 11 in, 2 out]
              }
              frame True {
              }
            }
            n129 = Strip Path(path=w222) -> (stripped path=w221:path)  [unwired: 1 out]
            n130 = Build Path(base path=w221, name or relative path="ActiveObjects_DynamicEvents_SubVIs") -> (appended path=w219:path)
            n131 = Bundle By Name(cluster=w226, "Data"=w225, "ClassType"=w196, "ClassFolder"=w223, "SupportFolder"=w219, "ProtectedFolder"=w217, "Application"=w212) -> (w229:T4)
          }
          frame "GetClassInfo" {
            n132 = call "GDSLvClass_GetClassProviderInformation.vi"("Class Refnum In"=w284, "error in (no error)"=w283) -> ("Class Refnum Out"=w276:refnum<vi>, "ClassProvider"=w278:T3, "error out"=w275:errorcluster)  [unwired: 15 in]
            n133 = call "GDSLvClass_ReadClassType.vi"("Class Refnum In"=w276, "error in (no error)"=w275) -> ("ClassSettings"=w273:T15, "error out"=w274:errorcluster)  [unwired: 15 in, 1 out]
            n134 = case shown="\"EndevoGOOP3\", \"EndevoGOOP4\"" w278 {
              tunnel: ["ActiveObjects_DynamicEvents_ProcessRepository_Native.vi" ("name or relative path") "ActiveObjects_DynamicEvents_ProcessRepository_EndevoGoop3.vi" ("name or relative path")] -> w281
              frame "Native", Default {
              }
              frame "EndevoGOOP3", "EndevoGOOP4" {
              }
            }
            n135 = Unbundle By Name(w273) -> ("ClassTemplateUsed"=w272:string)
            n136 = Unbundle By Name(w280) -> ("SupportFolder"=w282:path)
            n137 = Build Path(base path=w282, name or relative path=w281) -> (appended path=w279:path)
            n138 = Bundle By Name(cluster=w280, "ProcessRepository"=w279, "ClassProvider"=w278, "TemplateName"=w272) -> (w277:T4)
          }
          frame "CreateProcessCtlFile" {
            n139 = Unbundle By Name(w298) -> ("ProtectedFolder"=w293:refnum<vi>, "ClassFolder"=w311:path, "Data.ProcessName"=w310:string)
            n140 = Unbundle By Name(w298) -> ("SupportFolder"=w303:path, "Application"=w292:refnum<vi>)
            n141 = Concatenate Strings(w310, ".ctl" ("string")) -> (w308:string)
            n142 = Build Path(base path=w303, name or relative path="ActiveObjects_DynamicEvents_Process.ctl") -> (appended path=w290:path)
            n143 = Build Path(base path=w311, name or relative path=w308) -> (appended path=w300:path)
            n144 = New VI(8:w307, 9:T10."Control VI" ("vi type (standard vi)"), 10:w290, 11:w292) -> (0:w304:errorcluster, 3:w305:refnum<vi>)  [unwired: 3 in]
            n145 = invoke class="VI" method="Save.Instrument"(reference=w305, error in=w304, "Path to saved file"=w300) -> (reference out=w299:refnum<vi>, error out=w301:errorcluster)  [unwired: 3 in, 4 out]
            n146 = invoke class="ProjectItem" method="AddFile"(reference=w293, error in=w301, "Path"=w300) -> (error out=w289:errorcluster, "AddFile"=w291:refnum<vi>)  [unwired: 1 in, 2 out]
            n147 = call "CommonVIs_Wait.vi"("error in"=w289) -> ("error out"=w288:errorcluster)  [unwired: 9 in]
            n148 = Close Reference(reference=w291, error in (no error)=w288) -> ()  [unwired: 1 out]
            n149 = invoke class="VI" method="Save.Instrument"(reference=w299, error in=w288) -> (reference out=w296:refnum<vi>, error out=w294:errorcluster)  [unwired: 4 in, 4 out]
            n150 = Bundle By Name(cluster=w298, "ProcessCtl"=w296) -> (w297:T4)
          }
          frame "CreateProcessVI" {
            n151 = Unbundle By Name(w322) -> ("SupportFolder"=w327:path, "Application"=w316:refnum<vi>)
            n152 = Unbundle By Name(w322) -> ("ProtectedFolder"=w317:refnum<vi>, "ClassFolder"=w335:path, "Data.ProcessName"=w334:string)
            n153 = Concatenate Strings(w334, ".vi" ("string")) -> (w332:string)
            n154 = Build Path(base path=w327, name or relative path="ActiveObjects_DynamicEvents_Process.vi") -> (appended path=w314:path)
            n155 = Build Path(base path=w335, name or relative path=w332) -> (appended path=w324:path)
            n156 = New VI(8:w331, 9:T10."Standard VI" ("vi type (standard vi)"), 10:w314, 11:w316) -> (0:w328:errorcluster, 3:w329:refnum<vi>)  [unwired: 3 in]
            n157 = invoke class="VI" method="Save.Instrument"(reference=w329, error in=w328, "Path to saved file"=w324) -> (reference out=w323:refnum<vi>, error out=w325:errorcluster)  [unwired: 3 in, 4 out]
            n158 = invoke class="ProjectItem" method="AddFile"(reference=w317, error in=w325, "Path"=w324) -> (error out=w313:errorcluster, "AddFile"=w315:refnum<vi>)  [unwired: 1 in, 2 out]
            n159 = call "CommonVIs_Wait.vi"("error in"=w313) -> ("error out"=w312:errorcluster)  [unwired: 9 in]
            n160 = Close Reference(reference=w315, error in (no error)=w312) -> ()  [unwired: 1 out]
            n161 = invoke class="VI" method="Save.Instrument"(reference=w323, error in=w312) -> (reference out=w320:refnum<vi>, error out=w318:errorcluster)  [unwired: 4 in, 4 out]
            n162 = Bundle By Name(cluster=w322, "VI_ToFindSingleton"=w314, "ProcessVI"=w320) -> (w321:T4)
          }
          frame "CreateStartProcessVI" {
            n163 = Unbundle By Name(w338) -> ("SupportFolder"=w352:path, "Application"=w342:refnum<vi>, "Data.ProcessCreation"=w341:T1)
            n164 = Unbundle By Name(w338) -> ("ProtectedFolder"=w343:refnum<vi>, "ClassFolder"=w360:path, "Data.StartName"=w359:string)
            n165 = case shown="\"Create one process per object instance\", Default" w341 {
              tunnel: ["ActiveObjects_DynamicEvents_StartProcess_OnePerObject.vi" ("name or relative path") "ActiveObjects_DynamicEvents_StartProcess_OnePerClass.vi" ("name or relative path")] -> w340
              frame "Create one process per object instance", Default {
              }
              frame "Create only one process for this class" {
              }
            }
            n166 = Concatenate Strings(w359, ".vi" ("string")) -> (w357:string)
            n167 = Build Path(base path=w352, name or relative path=w340) -> (appended path=w351:path)
            n168 = Build Path(base path=w360, name or relative path=w357) -> (appended path=w349:path)
            n169 = New VI(8:w356, 9:T10."Standard VI" ("vi type (standard vi)"), 10:w351, 11:w342) -> (0:w353:errorcluster, 3:w354:refnum<vi>)  [unwired: 3 in]
            n170 = invoke class="VI" method="Save.Instrument"(reference=w354, error in=w353, "Path to saved file"=w349) -> (reference out=w348:refnum<vi>, error out=w350:errorcluster)  [unwired: 3 in, 4 out]
            n171 = invoke class="ProjectItem" method="AddFile"(reference=w343, error in=w350, "Path"=w349) -> (error out=w337:errorcluster, "AddFile"=w339:refnum<vi>)  [unwired: 1 in, 2 out]
            n172 = call "CommonVIs_Wait.vi"("error in"=w337) -> ("error out"=w336:errorcluster)  [unwired: 9 in]
            n173 = Close Reference(reference=w339, error in (no error)=w336) -> ()  [unwired: 1 out]
            n174 = invoke class="VI" method="Save.Instrument"(reference=w348, error in=w336) -> (reference out=w346:refnum<vi>, error out=w344:errorcluster)  [unwired: 4 in, 4 out]
            n175 = Bundle By Name(cluster=w338, "StartVI"=w346) -> (w347:T4)
          }
          frame "CreateStopProcessVI" {
            n176 = Unbundle By Name(w367) -> ("ProtectedFolder"=w371:refnum<vi>, "ClassFolder"=w387:path, "Data.StopName"=w386:string)
            n177 = Unbundle By Name(w367) -> ("SupportFolder"=w379:path, "Application"=w370:refnum<vi>)  [unwired: 1 out]
            n178 = Unbundle By Name(w367) -> ("Data.AddWindowControlVI"=w366:bool)
            n179 = Concatenate Strings(w386, ".vi" ("string")) -> (w384:string)
            n180 = Build Path(base path=w379, name or relative path="ActiveObjects_DynamicEvents_StopProcess.vi") -> (appended path=w378:path)
            n181 = Build Path(base path=w387, name or relative path=w384) -> (appended path=w376:path)
            n182 = New VI(8:w383, 9:T10."Standard VI" ("vi type (standard vi)"), 10:w378, 11:w370) -> (0:w380:errorcluster, 3:w381:refnum<vi>)  [unwired: 3 in]
            n183 = invoke class="VI" method="Save.Instrument"(reference=w381, error in=w380, "Path to saved file"=w376) -> (reference out=w375:refnum<vi>, error out=w377:errorcluster)  [unwired: 3 in, 4 out]
            n184 = case shown="True" w366 {
              tunnel: ["CreateProcessRepositoryVI" "CreateWindowControlVI"] -> w365
              frame False {
              }
              frame True {
              }
            }
            n185 = invoke class="ProjectItem" method="AddFile"(reference=w371, error in=w377, "Path"=w376) -> (error out=w364:errorcluster, "AddFile"=w369:refnum<vi>)  [unwired: 1 in, 2 out]
            n186 = call "CommonVIs_Wait.vi"("error in"=w364) -> ("error out"=w363:errorcluster)  [unwired: 9 in]
            n187 = Close Reference(reference=w369, error in (no error)=w363) -> ()  [unwired: 1 out]
            n188 = invoke class="VI" method="Save.Instrument"(reference=w375, error in=w363) -> (reference out=w373:refnum<vi>, error out=w372:errorcluster)  [unwired: 4 in, 4 out]
            n189 = Bundle By Name(cluster=w367, "StopVI"=w373) -> (w374:T4)
          }
          frame "CreateWindowControlVI" {
            n190 = Unbundle By Name(w402) -> ("ClassFolder"=w416:path, "Data.WindowControlName"=w415:string)  [unwired: 1 out]
            n191 = Unbundle By Name(w402) -> ("SupportFolder"=w408:path, "Application"=w398:refnum<vi>, "ClassType"=w395:T9)
            n192 = To More Generic Class(target class=refnum<vi> refnum ("AddItem"), reference=w393) -> (generic class reference=w392:refnum<vi>)
            n193 = case shown="\"6x8x6_Singleton\"" w395 {
              tunnel: ["ActiveObjects_DynamicEvents_ControlWindow_4x4x4.vi" ("name or relative path") "ActiveObjects_DynamicEvents_ControlWindow_5x6x5.vi" ("name or relative path") "ActiveObjects_DynamicEvents_ControlWindow_6x8x6.vi" ("name or relative path") "ActiveObjects_DynamicEvents_ControlWindow_4x4x4_Singleton.vi" ("name or relative path") "ActiveObjects_DynamicEvents_ControlWindow_5x6x5_Singleton.vi" ("name or relative path") "ActiveObjects_DynamicEvents_ControlWindow_6x8x6_Singleton.vi" ("name or relative path")] -> w407
              frame "4x4x4", Default {
              }
              frame "5x6x5" {
              }
              frame "6x8x6" {
              }
              frame "4x4x4_Singleton" {
              }
              frame "5x6x5_Singleton" {
              }
              frame "6x8x6_Singleton" {
              }
            }
            n194 = Concatenate Strings(w415, ".vi" ("string")) -> (w413:string)
            n195 = Build Path(base path=w408, name or relative path=w407) -> (appended path=w406:path)
            n196 = Build Path(base path=w416, name or relative path=w413) -> (appended path=w404:path)
            n197 = New VI(8:w412, 9:T10."Standard VI" ("vi type (standard vi)"), 10:w406, 11:w398) -> (0:w409:errorcluster, 3:w410:refnum<vi>)  [unwired: 3 in]
            n198 = invoke class="VI" method="Save.Instrument"(reference=w410, error in=w409, "Path to saved file"=w404) -> (reference out=w403:refnum<vi>, error out=w405:errorcluster)  [unwired: 3 in, 4 out]
            n199 = invoke class="ProjectItem" method="AddFile"(reference=w392, error in=w405, "Path"=w404) -> (error out=w391:errorcluster, "AddFile"=w397:refnum<vi>)  [unwired: 1 in, 2 out]
            n200 = call "CommonVIs_Wait.vi"("error in"=w391) -> ("error out"=w390:errorcluster)  [unwired: 9 in]
            n201 = Close Reference(reference=w397, error in (no error)=w390) -> ()  [unwired: 1 out]
            n202 = invoke class="VI" method="Save.Instrument"(reference=w403, error in=w390) -> (reference out=w400:refnum<vi>, error out=w399:errorcluster)  [unwired: 4 in, 4 out]
            n203 = Bundle By Name(cluster=w402, "WindowControlVI"=w400) -> (w401:T4)
          }
          frame "CreateProcessRepositoryVI" {
            n204 = Unbundle By Name(w426) -> ("ClassProvider"=w425:T3)
            n205 = Unbundle By Name(w426) -> ("ProcessRepository"=w427:path, "Application"=w433:refnum<vi>)
            n206 = Unbundle By Name(w426) -> ("ProtectedFolder"=w434:refnum<vi>, "ClassFolder"=w445:path, "Data.ProcessName"=w432:string)
            n207 = Format Into String(format string="%sRepository.vi", w432) -> (resulting string=w430:string)  [unwired: 2 in, 1 out]
            n208 = New VI(8:w444, 9:T10."Standard VI" ("vi type (standard vi)"), 10:w427, 11:w433) -> (0:w441:errorcluster, 3:w442:refnum<vi>)  [unwired: 3 in]
            n209 = Build Path(base path=w445, name or relative path=w430) -> (appended path=w439:path)
            n210 = invoke class="VI" method="Save.Instrument"(reference=w442, error in=w441, "Path to saved file"=w439) -> (reference out=w438:refnum<vi>, error out=w440:errorcluster)  [unwired: 3 in, 4 out]
            n211 = invoke class="ProjectItem" method="AddFile"(reference=w434, error in=w440, "Path"=w439) -> (error out=w424:errorcluster, "AddFile"=w429:refnum<vi>)  [unwired: 1 in, 2 out]
            n212 = case shown="Default" w425 {
              tunnel: ["UpdateOORefInVIs" "AddCtlToAttribute"] -> w428
              frame Default {
              }
              frame "UnKnown(LabVOOP)", "Native" {
              }
            }
            n213 = call "CommonVIs_Wait.vi"("error in"=w424) -> ("error out"=w423:errorcluster)  [unwired: 9 in]
            n214 = Close Reference(reference=w429, error in (no error)=w423) -> ()  [unwired: 1 out]
            n215 = invoke class="VI" method="Save.Instrument"(reference=w438, error in=w423) -> (reference out=w436:refnum<vi>, error out=w435:errorcluster)  [unwired: 4 in, 4 out]
            n216 = Bundle By Name(cluster=w426, "RepositoryVI"=w436) -> (w437:T4)
          }
          frame "AddCtlToAttribute" {
            w448 = T20[] [enum."UINT32"] items=["UINT8", "INT8", "UINT16", "INT16", "UINT32", "INT32", "UINT64", "INT64", "SGL", "DBL", "EXT", "CSG", "CDB", "CXT", "TimeStamp", "STRING", "PATH", "BOOL", "ENUM", "RefNum", "VIRefNum", "LabVIEW Class", "Cluster", "Variant", "TypeDef", "Waveform", "LabVIEW Object", "Other", "void", "Set", "Map"] ("DataTypes")
            n217 = call "Scripting_PlaceControlsInClassAttribute.vi"("ClassRefnum"=w452, "DeleteAllCurrentAttributesFirst(True)"=FALSE, "ControlNames"=string[] ["ProcessId:Process#No"], "DataTypes"=w448, "error in"=w460, "DeleteReferencesToCreatedAttributes(True)"=FALSE) -> ("ControlsCreated"=w456:refnum<vi>[], "error out"=w451:errorcluster)  [unwired: 7 in, 1 out]
            n218 = Index Array(array=w456) -> (element=w453:refnum<vi>)  [unwired: 1 in]
            n219 = call "GDSLvClass_SaveEverythingInClass.vi"("ClassRefIn"=w452, "error in"=w451) -> ("error out"=w450:errorcluster)  [unwired: 16 in, 1 out]
            n220 = Bundle By Name(cluster=w455, "ProcessIdRef"=w453) -> (w454:T4)
          }
          frame "UpdateOORefInVIs" {
            n221 = Unbundle By Name(w475) -> ("Data.AddWindowControlVI"=w461:bool, "ProcessVI"=w474:refnum<vi>, "StartVI"=w473:refnum<vi>, "StopVI"=w472:refnum<vi>, "RepositoryVI"=w464:refnum<vi>, "WindowControlVI"=w462:refnum<vi>, "ClassProvider"=w463:T3)
            n222 = property class="LVClassLibrary"(reference=w470) -> ("Path"=w466:path)  [unwired: 1 in, 2 out]
            n223 = case shown="False" w461 {
              tunnel: w474 -> [w481 w486]
              tunnel: w473 -> [w480 w485]
              tunnel: w472 -> [w479 w484]
              tunnel: [w478 w483] -> w469
              tunnel: w464 -> [w477 w482]
              tunnel: w462 -> [w476 _]
              frame True {
                n224 = Build Array(w481, w480, w479, w477, w476) -> (w478:refnum<vi>[])
              }
              frame False {
                n225 = Build Array(w486, w485, w484, w482) -> (w483:refnum<vi>[])
              }
            }
            n226 = Path To String(path=w466) -> (string=w465:string)
            n227 = for {
              tunnel: w469 -> [w489] mode=indexing
              shift-right: [w492] -> w468
              shift-left: w471 -> [w491]
              tunnel: w465 -> [w490]
              n228 = call "Scripting_ReplaceOORef.vi"("ViRef"=w489, "NewLvClassFile(ProjectPath or LvClassPath)"=w490, "error in (no error)"=w491) -> ("error out"=w492:errorcluster)  [unwired: 16 in]
            }
            n229 = case shown="Default" w463 {
              tunnel: ["UpdateVIs" "RenameProcessIdControl"] -> w467
              frame Default {
              }
              frame "UnKnown(LabVOOP)", "Native" {
              }
            }
          }
          frame "RenameProcessIdControl" {
            w493 = T20[] [enum."UINT32"] items=["UINT8", "INT8", "UINT16", "INT16", "UINT32", "INT32", "UINT64", "INT64", "SGL", "DBL", "EXT", "CSG", "CDB", "CXT", "TimeStamp", "STRING", "PATH", "BOOL", "ENUM", "RefNum", "VIRefNum", "LabVIEW Class", "Cluster", "Variant", "TypeDef", "Waveform", "LabVIEW Object", "Other", "void", "Set", "Map"] ("DataTypes")
            n230 = Unbundle By Name(w509) -> ("ProcessIdRef"=w512:refnum<vi>, "Data.ProcessName"=w507:string)
            n231 = Format Into String(format string="ProcessId:%s", w507) -> (resulting string=w506:string)  [unwired: 2 in, 1 out]
            n232 = property class="Ctl"(reference=w512, error in=w511, "Label.Text"=w506) -> (error out=w502:errorcluster)  [unwired: 1 out]
            n233 = call "Scripting_PlaceControlsInClassAttribute.vi"("ClassRefnum"=w500, "DeleteAllCurrentAttributesFirst(True)"=FALSE, "ControlNames"=string[] ["DummyStringThatShouldBeDeleted"], "DataTypes"=w493, "error in"=w502, "DeleteReferencesToCreatedAttributes(True)"=FALSE) -> ("ControlsCreated"=w499:refnum<vi>[], "error out"=w501:errorcluster)  [unwired: 7 in, 1 out]
            n234 = Index Array(array=w499) -> (element=w498:refnum<vi>)  [unwired: 1 in]
            n235 = call "GDSLvClass_SaveEverythingInClass.vi"("ClassRefIn"=w500, "ForceResaving(False)"=TRUE, "error in"=w501) -> ("ClassRefOut"=w496:refnum<vi>, "error out"=w495:errorcluster)  [unwired: 15 in]
            n236 = invoke class="Ctl" method="Delete"(reference=w498, error in=w495) -> (error out=w497:errorcluster)  [unwired: 1 in, 2 out]
            n237 = call "GDSLvClass_SaveEverythingInClass.vi"("ClassRefIn"=w496, "error in"=w497) -> ("error out"=w494:errorcluster)  [unwired: 16 in, 1 out]
          }
          frame "UpdateVIs" {
            n238 = vi-ref "JKI_Copy_Parse State Queue.vi"() -> (w528:refnum<vi>)
            n239 = Unbundle By Name(w533) -> ("Data.AddWindowControlVI"=w530:bool, "ProcessVI"=w543:refnum<vi>, "StartVI"=w542:refnum<vi>, "StopVI"=w541:refnum<vi>, "WindowControlVI"=w531:refnum<vi>, "RepositoryVI"=w537:refnum<vi>)
            n240 = Unbundle By Name(w533) -> ("SupportFolder"=w523:path)
            n241 = Unbundle By Name(w533) -> ("RepositoryVI"=w551:refnum<vi>, "ProcessCtl"=w546:refnum<vi>)
            n242 = vi-ref "JKI_Copy_Add State(s) to Queue.vi"() -> (w526:refnum<vi>)
            n243 = property class="VI"(reference=w528) -> ("Path"=w527:path)  [unwired: 1 in, 2 out]
            n244 = property class="VI"(reference=w526) -> ("Path"=w525:path)  [unwired: 1 in, 2 out]
            n245 = Unbundle By Name(w533) -> ("SupportFolder"=w550:path)
            n246 = VI Library() -> (path=w514:path)
            n247 = case shown="False" w530 {
              tunnel: w543 -> [w569 w573]
              tunnel: w542 -> [w568 w572]
              tunnel: w541 -> [w567 w571]
              tunnel: [w566 w570] -> w538
              tunnel: w531 -> [w565 _]
              frame True {
                n248 = Build Array(w569, w568, w567, w565) -> (w566:refnum<vi>[])
              }
              frame False {
                n249 = Build Array(w573, w572, w571) -> (w570:refnum<vi>[])
              }
            }
            n250 = property class="VI"(reference=w546) -> ("Path"=w545:path)  [unwired: 1 in, 2 out]
            n251 = Build Path(base path=w514, name or relative path=path "addons/_JKI Toolkits/State Machine/_JKI_lib_State_Machine.llb") -> (appended path=w517:path)
            n252 = property class="VI"(reference=w537) -> ("Path"=w536:path)  [unwired: 1 in, 2 out]
            n253 = Build Path(base path=w550, name or relative path="ActiveObjects_DynamicEvents_Process.ctl") -> (appended path=w548:path)
            n254 = Build Path(base path=w517, name or relative path=path "Parse State Queue__jki_lib_state_machine.vi") -> (appended path=w520:path)
            n255 = Build Path(base path=w517, name or relative path=path "Add State(s) to Queue__jki_lib_state_machine.vi") -> (appended path=w515:path)
            n256 = Build Path(base path=w523, name or relative path="ActiveObjects_DynamicEvents_ProcessRepository_Native.vi") -> (appended path=w532:path)
            n257 = Build Array(w548) -> (w547:path[])
            n258 = Build Array(w545) -> (w544:path[])
            n259 = call <vilib>:"Check if File or Folder Exists.vi"("path"=w520) -> ("file or folder exists?"=w519:bool, "dup path"=w518:path)  [unwired: 8 in, 1 out]
            n260 = case shown="True" w519 {
              tunnel: w536 -> [w560 w564]
              tunnel: [w559 w563] -> w535
              tunnel: [w558 w562] -> w534
              tunnel: w532 -> [w557 w561]
              tunnel: w527 -> [w556 _]
              tunnel: w525 -> [w555 _]
              tunnel: w518 -> [w554 _]
              tunnel: w515 -> [w553 _]
              frame True {
                n261 = Build Array(w557, w556, w555) -> (w558:path[])
                n262 = Build Array(w560, w554, w553) -> (w559:path[])
              }
              frame False {
                n263 = Build Array(w564) -> (w563:path[])
                n264 = Build Array(w561) -> (w562:path[])
              }
            }
            n265 = call "Scripting_ReplaceVisAndControls.vi"("ViRef"=w551, "OldVIsAndControls"=w547, "NewVIsAndControls"=w544, "error in (no error)"=w529) -> ("error out"=w540:errorcluster)  [unwired: 14 in, 1 out]
            n266 = for {
              shift-right: [w577] -> w539
              shift-left: w540 -> [w578]
              tunnel: w538 -> [w576] mode=indexing
              tunnel: w535 -> [w575]
              tunnel: w534 -> [w574]
              n267 = call "Scripting_ReplaceVisAndControls.vi"("ViRef"=w576, "OldVIsAndControls"=w574, "NewVIsAndControls"=w575, "error in (no error)"=w578) -> ("error out"=w577:errorcluster)  [unwired: 14 in, 1 out]
            }
          }
          frame "UpdateRepositoryStaticVI" {
            (unwired) T9."6x8x6_Singleton" ("ClassType")
            (unwired) T9."4x4x4_Singleton" ("ClassType")
            w592 = refnum<vi> refnum  # StaticVIReference
            n268 = Unbundle By Name(w580) -> ("RepositoryVI"=w596:refnum<vi>)
            n269 = Unbundle By Name(w580) -> ("ClassType"=w579:T9)
            n270 = Unbundle By Name(w580) -> ("ClassFolder"=w585:path, "Data.ProcessName"=w584:string)
            n271 = Concatenate Strings(w584, ".vi" ("string")) -> (w582:string)
            n272 = Build Path(base path=w585, name or relative path=w582) -> (appended path=w581:path)
            n273 = call "Scripting_FindNodeOnDiagram.vi"("ViRef(Ignored If Not Wired)"=w596, "NodeTypesToSearchFor"=string[] ["StaticVIReference"], "error in (no error)"=w595) -> ("Nodes"=w588:refnum<vi>[], "error out"=w587:errorcluster)  [unwired: 15 in]
            n274 = Index Array(array=w588) -> (element=w593:refnum<vi>)  [unwired: 1 in]
            n275 = To More Specific Class(target class=w592, reference=w593, error in=w587) -> (specific class reference=w591:refnum<vi>, error out=w590:errorcluster)
            n276 = property class="StatVIRef"(reference=w591, error in=w590, "Path"=w581) -> (error out=w589:errorcluster)  [unwired: 1 out]
            n277 = case shown="\"4x4x4_Singleton\"..\"6x8x6_Singleton\"" w579 {
              tunnel: ["FixViRefType" "FixSingletonCodeWithGetInstance"] -> w597
              frame Default {
              }
              frame "4x4x4_Singleton".."6x8x6_Singleton" {
              }
            }
            n278 = Close Reference(reference=w588, error in (no error)=w589) -> (error out=w586:errorcluster)
          }
          frame "FixSingletonCodeWithGetInstance" {
            n279 = Unbundle By Name(w605) -> ("VI_ToFindSingleton"=w611:path, "WindowControlVI"=w603:refnum<vi>)
            n280 = call "GDSLvClass_GetClassMethod.vi"("Class Refnum In"=w606, "VINames"=string[] ["GetInstance.vi$"] ("VIsToSerachFor/ViName"), "error in (no error)"=w609) -> ("ViPaths"=w604:path[], "error out"=w612:errorcluster)  [unwired: 13 in, 2 out]
            n281 = Empty Array?(array=w604) -> (empty?=w601:bool)
            n282 = Not A Number/Path/Refnum?(number/path/refnum=w603) -> (NaN/Path/Refnum?=w602:bool)
            n283 = Build Array(w611) -> (w610:path[])
            n284 = Or(x=w602, y=w601) -> (x .or. y?=w600:bool)
            n285 = case shown="False" w600 {
              tunnel: w612 -> [w620 w625]
              tunnel: w610 -> [w619 _]
              tunnel: [w616 w625] -> w608
              tunnel: w604 -> [w615 _]
              tunnel: w603 -> [w614 _]
              frame False {
                n286 = call "Scripting_FindVisOnDiagram.vi"("ViRef"=w614, "VIsToSerachFor/ViName"=w619, "error in (no error)"=w620) -> ("VisFound"=w622:refnum<vi>[], "error out"=w621:errorcluster)  [unwired: 15 in]
                n287 = Index Array(array=w615) -> (element=w618:path)  [unwired: 1 in]
                n288 = Index Array(array=w622) -> (element=w623:refnum<vi>)  [unwired: 1 in]
                n289 = invoke class="GObj" method="Replace"(reference=w623, error in=w621, "Path"=w618) -> (error out=w617:errorcluster, "Replace"=w624:refnum<vi>)  [unwired: 3 in, 4 out]
                n290 = Close Reference(reference=w622, error in (no error)=w617) -> ()  [unwired: 1 out]
                n291 = Close Reference(reference=w624, error in (no error)=w617) -> (error out=w616:errorcluster)
              }
              frame True {
              }
            }
          }
          frame "FixViRefType" {
            w639 = refnum<vi> refnum  # VIRefNum
            w654 = refnum<vi> refnum  # VIRefNum
            w662 = refnum<vi> refnum  # Cluster
            n292 = Unbundle By Name(w665) -> ("ProcessCtl"=w627:refnum<vi>, "RepositoryVI"=w626:refnum<vi>, "ProcessVI"=w637:refnum<vi>)
            n293 = property class="VI"(reference=w627, error in=w630) -> (reference out=w650:refnum<vi>, error out=w660:errorcluster, "Panel"=w664:refnum<vi>)
            n294 = property class="Pnl"(reference=w664, error in=w660) -> (reference out=w649:refnum<vi>, error out=w661:errorcluster, "Controls[]"=w648:refnum<vi>[])
            n295 = Index Array(array=w648) -> (element=w663:refnum<vi>)  [unwired: 1 in]
            n296 = To More Specific Class(target class=w662, reference=w663, error in=w661) -> (specific class reference=w659:refnum<vi>, error out=w658:errorcluster)
            n297 = property class="Clust"(reference=w659, error in=w658) -> (error out=w655:errorcluster, "Controls[]"=w657:refnum<vi>[])  [unwired: 1 out]
            n298 = Index Array(array=w657, index=3) -> (element=w629:refnum<vi>)
            n299 = To More Specific Class(target class=w654, reference=w629, error in=w655) -> (specific class reference=w653:refnum<vi>, error out=w652:errorcluster)
            n300 = invoke class="VIRef" method="Make Strict Reference"(reference=w653, error in=w652, "VI Ref"=w637) -> (error out=w651:errorcluster)  [unwired: 1 in, 3 out]
            n301 = invoke class="VI" method="Save.Instrument"(reference=w650, error in=w651) -> (error out=w632:errorcluster)  [unwired: 4 in, 5 out]
            n302 = property class="VI"(reference=w626, error in=w632) -> (reference out=w636:refnum<vi>, error out=w646:errorcluster, "Panel"=w645:refnum<vi>)
            n303 = property class="Pnl"(reference=w645, error in=w646) -> (reference out=w633:refnum<vi>, error out=w643:errorcluster, "Controls[]"=w635:refnum<vi>[])
            n304 = for {
              tunnel: w635 -> [w673] mode=indexing
              tunnel: "ProcessViRef" -> [w672]
              shift-right: [w668] -> w638
              shift-left: w643 -> [w669]
              tunnel: [w667] -> w628
              stop <- w670 stop-if-true
              n305 = property class="Ctl"(reference=w673, error in=w669) -> (reference out=w667:refnum<vi>, error out=w668:errorcluster, "Label.Text"=w671:string)
              n306 = Equal?(x=w671, y=w672) -> (x = y?=w670:bool)
            }
            n307 = To More Specific Class(target class=w639, reference=w628, error in=w638) -> (specific class reference=w640:refnum<vi>, error out=w641:errorcluster)
            n308 = invoke class="VIRef" method="Make Strict Reference"(reference=w640, error in=w641, "VI Ref"=w637) -> (error out=w642:errorcluster)  [unwired: 1 in, 3 out]
            n309 = invoke class="VI" method="Save.Instrument"(reference=w636, error in=w642) -> (error out=w631:errorcluster)  [unwired: 4 in, 5 out]
            n310 = Close Reference(reference=w635, error in (no error)=w631) -> (error out=w634:errorcluster)
            n311 = Close Reference(reference=w633, error in (no error)=w634) -> ()  [unwired: 1 out]
            n312 = Close Reference(reference=w648, error in (no error)=w632) -> (error out=w647:errorcluster)
            n313 = Close Reference(reference=w649, error in (no error)=w647) -> ()  [unwired: 1 out]
          }
          frame "UpdateIcons" {
            w710 = u8 32 ("x")
            n314 = Unbundle By Name(w689) -> ("Data.AddWindowControlVI"=w675:bool, "ProcessVI"=w692:refnum<vi>, "StartVI"=w691:refnum<vi>, "StopVI"=w690:refnum<vi>, "RepositoryVI"=w681:refnum<vi>, "WindowControlVI"=w677:refnum<vi>, "Data.ProcessName"=w680:string, "Data.StartName"=w684:string, "Data.StopName"=w683:string, "Data.WindowControlName"=w676:string)
            n315 = property class="LVClassLibrary"(reference=w693, error in=w687) -> (reference out=w698:refnum<vi>, error out=w694:errorcluster, "Member Data"=w696:refnum<vi>)
            n316 = call "GDSLvIcon_AnalyseViIcon.vi"("ViRef/LvCLassRef/LvLibRef/ViPath/2D_Image"=w696, "error in (no error)"=w694) -> ("HeaderIcon"=w699:u8[][], "error out"=w695:errorcluster)  [unwired: 5 in, 11 out]
            n317 = case shown="True" w675 {
              tunnel: w692 -> [w720 w725]
              tunnel: w691 -> [w719 w724]
              tunnel: w690 -> [w718 w723]
              tunnel: [w717 w722] -> w685
              tunnel: w681 -> [w716 w721]
              tunnel: w677 -> [w715 _]
              frame True {
                n318 = Build Array(w720, w719, w718, w716, w715) -> (w717:refnum<vi>[])
              }
              frame False {
                n319 = Build Array(w725, w724, w723, w721) -> (w722:refnum<vi>[])
              }
            }
            n320 = Close Reference(reference=w696, error in (no error)=w695) -> (error out=w697:errorcluster)
            n321 = Format Into String(format string="%sRepository", w680) -> (resulting string=w679:string)  [unwired: 2 in, 1 out]
            n322 = Array Size(array=w699) -> (size(s)=w705:i32[])
            n323 = call "GDSLvClass_ReadClassColors.vi"("Library Refnum"=w698, "error in (no error)"=w697) -> ("LvClassIconSettings"=w701:T21, "error out"=w688:errorcluster)  [unwired: 12 in, 4 out]
            n324 = Unbundle By Name(w701) -> ("Frame"=w704:u32, "Body Text"=w703:u32, "Frame thickness"=w700:u8)
            n325 = Build Array(w680, w684, w683, w679, w676) -> (w682:string[])
            n326 = Unbundle By Name(w701) -> ("ColorPublic"=w674:u32, "ColorProtected"=w702:u32)
            n327 = Index Array(array=w705) -> (element #1=w707:i32)  [unwired: 2 in, 1 out]
            n328 = Multiply(x=w700, y=u8 2) -> (x*y=w708:u8)
            n329 = Add(x=w707, y=w708) -> (x+y=w709:i32)
            n330 = Increment(x=w709) -> (x+1=w711:i32)
            n331 = Subtract(x=w710, y=w711) -> (x-y=w712:i32)
            n332 = Subtract(x=w710, y=w708) -> (x-y=w713:u8)
            n333 = for {
              tunnel: w713 -> [w751]
              tunnel: w712 -> [w750]
              tunnel: w704 -> [w747]
              tunnel: w703 -> [w746]
              tunnel: w702 -> [w727]
              tunnel: w700 -> [w745]
              tunnel: w699 -> [w744]
              shift-right: [w734] -> w686
              shift-left: w688 -> [w736]
              tunnel: w685 -> [w733] mode=indexing
              tunnel: w682 -> [w732] mode=indexing
              tunnel: w674 -> [w728]
              i -> [w731]
              n334 = Bundle By Name(cluster=T11 {"Text"="", "Allow Only Capital Chars"=TRUE, "Compression"=enum."Auto", "Alignment"=enum."Center"} ("Text"), "Text"=w732) -> (w749:T11)
              n335 = Equal?(x=w731, y=4) -> (x = y?=w729:bool)
              n336 = Select(t=w728, s=w729, f=w727) -> (s? t:f=w726:u32)
              n337 = call "GDSLvIcon_GenerateIconText.vi"("Text"=w749, "TextPixelHeight(5-30)"=w750, "Foreground color"=w746, "Background color"=w726, "error in (no error)"=w736, "Text Pixel width(32-FrameThicknes*2))"=w751) -> ("TextOut"=w743:u8[][], "error out"=w735:errorcluster)  [unwired: 9 in, 3 out]
              n338 = call "GDSLvIcon_CreateIconPicture.vi"("FrameColor"=w747, "FrameThickness(1)"=w745, "HeaderIconIn"=w744, "BodyIconIn"=w743, "error in (no error)"=w735) -> ("WholeIconOut"=w738:u8[][], "error out"=w741:errorcluster)  [unwired: 9 in, 4 out]
              n339 = Reshape Array(w738, 1024 ("dimension size")) -> (w740:u8[])
              n340 = Bundle By Name(cluster=T14 {"image type"=0, "image depth"=8, "image"=[], "mask"=[], "colors"=[], "Rectangle"={"left"=0, "top"=0, "right"=32, "bottom"=32}} ("image data"), "image"=w740) -> (w742:T14)
              n341 = invoke class="VI" method="VI Icon.Set from Image Data"(reference=w733, error in=w741, "ImageData"=w742) -> (error out=w734:errorcluster)  [unwired: 3 in, 5 out]
            }
          }
          frame "UpdateCreate?" {
            n342 = Unbundle By Name(w753) -> ("Data.AddInConstructor"=w756:bool)
            n343 = case shown="True" w756 {
              tunnel: w757 -> [w758 w779]
              tunnel: [w758 w778] -> w755
              tunnel: w753 -> [_ w777]
              tunnel: w752 -> [_ w773]
              frame False {
              }
              frame True {
                n344 = Unbundle By Name(w777) -> ("Application"=w766:refnum<vi>, "StartVI"=w776:refnum<vi>, "ClassProvider"=w774:T3, "TemplateName"=w763:string)
                n345 = property class="LVClassLibrary"(reference=w773) -> ("Path"=w772:path)  [unwired: 1 in, 2 out]
                n346 = To Lower Case(string=w763) -> (all lower case string=w762:string)
                n347 = Strip Path(path=w772) -> (stripped path=w771:path)  [unwired: 1 out]
                n348 = Match Pattern(string=w762, regular expression="singleton") -> (offset past match=w760:i32)  [unwired: 1 in, 3 out]
                n349 = Greater Or Equal To 0?(x=w760) -> (x >= 0?=w759:bool)
                n350 = property class="VI"(reference=w776) -> ("Path"=w775:path)  [unwired: 1 in, 2 out]
                n351 = case shown="\"EndevoGOOP3\", \"EndevoGOOP4\"" w774 {
                  tunnel: ["*Init.vi" w800 "*_Create.vi" "Constructor*.vi"] -> w770
                  tunnel: w759 -> [_ w799 _ _]
                  frame "Native", Default {
                  }
                  frame "EndevoGOOP3", "EndevoGOOP4" {
                    n352 = case shown="True" w799 {
                      tunnel: ["*Init.vi" "*_Create.vi"] -> w800
                      frame True {
                      }
                      frame False {
                      }
                    }
                  }
                  frame "OpenG(RootObject)" {
                  }
                  frame "OpenG(OpenG_Object)" {
                  }
                }
                n353 = call <vilib>:"Recursive File List.vi"("pattern"=w770, "Treat LLBs as Folders?"=TRUE, "Folder Path"=w771) -> ("All Files in Dir"=w768:path[])  [unwired: 4 in, 4 out]
                n354 = Index Array(array=w768) -> (element=w765:path)  [unwired: 1 in]
                n355 = call <vilib>:"Check if File or Folder Exists.vi"("path"=w765) -> ("file or folder exists?"=w767:bool)  [unwired: 8 in, 2 out]
                n356 = case shown="True" w767 {
                  tunnel: w779 -> [w780 w781]
                  tunnel: [w780 w782] -> w778
                  tunnel: w775 -> [_ w793]
                  tunnel: w766 -> [_ w791]
                  tunnel: w765 -> [_ w790]
                  tunnel: "The \"Start Process VI\" could not automatically be placed in the Create/Construct method.\nPlease add this method manually." ("message") -> [_ w784]
                  frame False {
                  }
                  frame True {
                    n357 = Open VI Reference(application reference (local)=w791, vi path=w790, error in (no error)=w781) -> (vi reference=w789:refnum<vi>, error out=w792:errorcluster)  [unwired: 3 in]
                    n358 = call "Scripting_AddVIInsideNoErrorCase.vi"("ViToModify"=w789, "VIToAdd"=w793, "error in (no error)"=w792, "AddVIOnLeftSideCaseStructure"=FALSE, "OnlyReference"=FALSE) -> ("error out"=w788:errorcluster)  [unwired: 14 in]
                    n359 = invoke class="VI" method="Save.Instrument"(reference=w789, error in=w788) -> (reference out=w786:refnum<vi>, error out=w787:errorcluster)  [unwired: 4 in, 4 out]
                    n360 = Close Reference(reference=w786, error in (no error)=w787) -> (error out=w783:errorcluster)
                    n361 = case shown="Error" w783 {
                      selector: w783 -> [w795 _]
                      tunnel: [w795 w797] -> w782
                      tunnel: w781 -> [_ w797]
                      tunnel: w784 -> [_ w796]
                      frame No Error {
                      }
                      frame Error {
                        n362 = One Button Dialog(message=w796) -> ()  [unwired: 1 in, 1 out]
                      }
                    }
                  }
                }
              }
            }
          }
          frame "UpdateDestroy?" {
            n363 = Unbundle By Name(w806) -> ("Data.AddInDestructor"=w809:bool)
            n364 = case shown="True" w809 {
              tunnel: w810 -> [w811 w821]
              tunnel: [w811 w820] -> w808
              tunnel: w806 -> [_ w819]
              tunnel: w805 -> [_ w818]
              frame False {
              }
              frame True {
                n365 = Unbundle By Name(w819) -> ("Application"=w823:refnum<vi>, "StopVI"=w832:refnum<vi>, "ClassProvider"=w830:T3, "TemplateName"=w813:string)
                n366 = To Lower Case(string=w813) -> (all lower case string=w816:string)
                n367 = property class="LVClassLibrary"(reference=w818) -> ("Path"=w829:path)  [unwired: 1 in, 2 out]
                n368 = Strip Path(path=w829) -> (stripped path=w828:path)  [unwired: 1 out]
                n369 = Match Pattern(string=w816, regular expression="singleton") -> (offset past match=w814:i32)  [unwired: 1 in, 3 out]
                n370 = Greater Or Equal To 0?(x=w814) -> (x >= 0?=w812:bool)
                n371 = case shown="\"EndevoGOOP3\", \"EndevoGOOP4\"" w830 {
                  tunnel: ["CleanUp.vi" w864 "Destroy.vi" "Destructor*.vi"] -> w827
                  tunnel: w812 -> [_ w863 _ _]
                  frame "Native", Default {
                  }
                  frame "EndevoGOOP3", "EndevoGOOP4" {
                    n372 = case shown="False" w863 {
                      tunnel: ["*CleanUp.vi" "Destroy.vi"] -> w864
                      frame True {
                      }
                      frame False {
                      }
                    }
                  }
                  frame "OpenG(RootObject)" {
                  }
                  frame "OpenG(OpenG_Object)" {
                  }
                }
                n373 = call <vilib>:"Recursive File List.vi"("pattern"=w827, "Treat LLBs as Folders?"=TRUE, "Folder Path"=w828) -> ("All Files in Dir"=w825:path[])  [unwired: 4 in, 4 out]
                n374 = property class="VI"(reference=w832) -> ("Path"=w831:path)  [unwired: 1 in, 2 out]
                n375 = Index Array(array=w825) -> (element=w822:path)  [unwired: 1 in]
                n376 = call <vilib>:"Check if File or Folder Exists.vi"("path"=w822) -> ("file or folder exists?"=w824:bool)  [unwired: 8 in, 2 out]
                n377 = case shown="True" w824 {
                  tunnel: w821 -> [w833 w836]
                  tunnel: [w833 w837] -> w820
                  tunnel: w831 -> [_ w846]
                  tunnel: w823 -> [_ w844]
                  tunnel: w822 -> [_ w843]
                  tunnel: "The \"Stop Process VI\" could not automatically be placed in the Destroy/Destruct method.\nPlease add this method manually before the object is destroyed." ("message") -> [_ w835]
                  tunnel: w812 -> [_ w834]
                  frame False {
                  }
                  frame True {
                    n378 = Open VI Reference(application reference (local)=w844, vi path=w843, error in (no error)=w836) -> (vi reference=w842:refnum<vi>, error out=w845:errorcluster)  [unwired: 3 in]
                    n379 = case shown="True" w834 {
                      tunnel: w846 -> [w851 w858]
                      tunnel: w845 -> [w850 w857]
                      tunnel: w842 -> [w849 w855]
                      tunnel: [w848 w856] -> w841
                      frame False {
                        n380 = call "Scripting_AddVIInsideNoErrorCase.vi"("ViToModify"=w849, "VIToAdd"=w851, "error in (no error)"=w850, "AddVIOnLeftSideCaseStructure"=TRUE, "OnlyReference"=TRUE) -> ("error out"=w848:errorcluster)  [unwired: 14 in]
                      }
                      frame True {
                        n381 = call "Scripting_AddVIBetweenVIs.vi"("ViToModify"=w855, "VIToAdd"=w858, "VIOne(Path,Name or NamePattern)"="GetInstance.vi" ("regular expression"), "VITwo(Path,Name or NamePattern), If Left/Right-string, it will be placed to the right or left of VIOne"="GetAttributes.vi" ("regular expression"), "error in (no error)"=w857) -> ("error out"=w856:errorcluster)  [unwired: 13 in, 1 out]
                      }
                    }
                    n382 = invoke class="VI" method="Save.Instrument"(reference=w842, error in=w841) -> (reference out=w839:refnum<vi>, error out=w840:errorcluster)  [unwired: 4 in, 4 out]
                    n383 = Close Reference(reference=w839, error in (no error)=w840) -> (error out=w838:errorcluster)
                    n384 = case shown="Error" w838 {
                      selector: w838 -> [w859 _]
                      tunnel: [w859 w861] -> w837
                      tunnel: w836 -> [_ w861]
                      tunnel: w835 -> [_ w860]
                      frame No Error {
                      }
                      frame Error {
                        n385 = One Button Dialog(message=w860) -> ()  [unwired: 1 in, 1 out]
                      }
                    }
                  }
                }
              }
            }
          }
          frame "SaveAll" {
            n386 = Unbundle By Name(w873) -> ("ProcessVI"=w871:refnum<vi>, "Data.ProcessCreation"=w872:T1)
            n387 = case shown="\"Create one process per object instance\", Default" w872 {
              tunnel: w871 -> [_ w882]
              tunnel: w869 -> [w878 w880]
              tunnel: [w878 w879] -> w870
              frame "Create one process per object instance", Default {
              }
              frame "Create only one process for this class" {
                n388 = property class="VI"(reference=w882, error in=w880, "Exec.IsReentrant"=FALSE ("Execution:Is Reentrant")) -> (error out=w879:errorcluster)  [unwired: 1 out]
              }
            }
            n389 = call "GDSLvClass_SaveEverythingInClass.vi"("ClassRefIn"=w875, "ForceResaving(False)"=TRUE, "error in"=w870) -> ("error out"=w876:errorcluster)  [unwired: 15 in, 1 out]
          }
        }
        n390 = Equal?(x=w166, y="Exit") -> (x = y?=w169:bool)
        n391 = Select(t="Error", s=w165, f=w166) -> (s? t:f=w170:string)
      }
    }
    frame "RemovePattern" {
    }
    frame "UpdatePattern" {
    }
    frame "CreatePatternMethod" {
      w891 = "Init"
      n392 = property class="VI"(error in=w890, "Front Panel.Open"=FALSE ("Front Panel Window:Open")) -> (error out=w892:errorcluster)  [unwired: 1 in, 1 out]
      n393 = while {
        shift-right: [w901] -> w885
        shift-left: w892 -> [w908]
        shift-right: [w906] -> _
        shift-left: w891 -> [w907]
        shift-right: [w894] -> _
        shift-left: _ -> [w900]
        tunnel: w888 -> [w899]
        tunnel: w886 -> [w898]
        tunnel: w887 -> [w897]
        tunnel: w889 -> [w896]
        shift-left: w891 -> [w895]
        stop <- w905 stop-if-true
        n394 = case shown="\"Init\"" w907 {
          tunnel: w908 -> [w937 w955 w977]
          tunnel: [w929 w954 w978] -> w901
          tunnel: [w927 "ReplaceProcessRepositoryVI" "Exit"] -> w902
          tunnel: w900 -> [_ w941 w980]
          tunnel: w899 -> [w938 _ _]
          tunnel: w898 -> [_ _ _]
          tunnel: w897 -> [w918 _ _]
          tunnel: w896 -> [w930 w956 w979]
          tunnel: w895 -> [_ _ _]
          tunnel: [w912 w941 w980] -> w894
          frame "Init" {
            n395 = Variant To Data(error in=w937, type=cluster{path, "VI":refnum<vi>, "Name":string} {path "", "VI"=refnum, "Name"=""} ("cluster"), Variant=w938) -> (data=w920:cluster{path, "VI":refnum<vi>, "Name":string}, error out=w922:errorcluster)
            n396 = Unbundle(w920) -> (w917:path, "VI"=w916:refnum<vi>, "Name"=w909:string)
            n397 = call "GDSLvClass_ReadClassType.vi"("Class Refnum In"=w930, "error in (no error)"=w922) -> ("ClassSettings"=w936:T15, "error out"=w929:errorcluster)  [unwired: 15 in, 1 out]
            n398 = Unbundle By Name(w936) -> ("ConnectorPanePattern"=w935:string, "ClassTemplateUsed"=w934:string)
            n399 = To Lower Case(string=w934) -> (all lower case string=w932:string)
            n400 = case shown="\"0\", Default" w935 {
              tunnel: ["4x4x4" "6x8x6"] -> _
              frame "0", Default {
              }
              frame "1", "2" {
              }
            }
            n401 = Match Pattern(string=w932, regular expression="singleton" ("search string")) -> (offset past match=w933:i32)  [unwired: 1 in, 3 out]
            n402 = Greater Or Equal To 0?(x=w933) -> (x >= 0?=w928:bool)
            n403 = Current VI's Path() -> (path=w925:path)
            n404 = Strip Path(path=w925) -> (stripped path=w924:path)  [unwired: 1 out]
            n405 = Build Path(base path=w924, name or relative path="ActiveObjects_DynamicEvents_SubVIs") -> (appended path=w915:path)
            n406 = Build Path(base path=w915, name or relative path="ActiveObjects_DynamicEvents_ProcessRepository_Native.vi") -> (appended path=w913:path)
            n407 = Build Path(base path=w915, name or relative path="ActiveObjects_DynamicEvents_Process.vi") -> (appended path=w910:path)
            n408 = Bundle By Name(cluster=w918, "MethodTemplate"=w917, "VI"=w916, "SupportFolder"=w915, "VI_ToFind"=w913, "VI_ToFindSingleton"=w910, "Name"=w909) -> (w912:T4)
            n409 = Select(t="Place_GetInstanceVI", s=w928, f="ReplaceProcessRepositoryVI") -> (s? t:f=w927:string)
          }
          frame "Place_GetInstanceVI" {
            n410 = Unbundle By Name(w941) -> ("VI_ToFindSingleton"=w946:path, "VI"=w942:refnum<vi>)
            n411 = Build Array(w946) -> (w945:path[])
            n412 = call "GDSLvClass_GetClassMethod.vi"("Class Refnum In"=w956, "VINames"=string[] ["GetInstance.vi$"] ("VIsToSerachFor/ViName"), "error in (no error)"=w955) -> ("ViPaths"=w952:path[], "error out"=w947:errorcluster)  [unwired: 13 in, 2 out]
            n413 = call "Scripting_FindVisOnDiagram.vi"("ViRef"=w942, "VIsToSerachFor/ViName"=w945, "error in (no error)"=w947) -> ("VisFound"=w949:refnum<vi>[], "error out"=w948:errorcluster)  [unwired: 15 in]
            n414 = Index Array(array=w952) -> (element=w944:path)  [unwired: 1 in]
            n415 = Index Array(array=w949) -> (element=w950:refnum<vi>)  [unwired: 1 in]
            n416 = invoke class="GObj" method="Replace"(reference=w950, error in=w948, "Path"=w944) -> (error out=w943:errorcluster, "Replace"=w951:refnum<vi>)  [unwired: 3 in, 4 out]
            n417 = Close Reference(reference=w949, error in (no error)=w943) -> ()  [unwired: 1 out]
            n418 = Close Reference(reference=w951, error in (no error)=w943) -> (error out=w954:errorcluster)
          }
          frame "ReplaceGetClassAttributes", Default {
            w964 = "Repository.vi$"
            n419 = Unbundle By Name(w980) -> ("VI_ToFind"=w970:path, "VI"=w966:refnum<vi>, "Name"=w965:string)
            n420 = Build Array(w970) -> (w969:path[])
            n421 = Concatenate Strings(w965, w964) -> (w963:string)
            n422 = Build Array(w963, w964) -> (w958:string[])
            n423 = call "GDSLvClass_GetClassMethod.vi"("Class Refnum In"=w979, "VINames"=w958, "error in (no error)"=w977) -> ("ViPaths"=w967:path[], "error out"=w968:errorcluster)  [unwired: 13 in, 2 out]
            n424 = Index Array(array=w967) -> (element #1=w960:path, element #2=w961:path)  [unwired: 2 in]
            n425 = Empty String/Path?(string/path=w960) -> (empty?=w962:bool)
            n426 = Select(t=w961, s=w962, f=w960) -> (s? t:f=w959:path)
            n427 = call "Scripting_FindVisOnDiagram.vi"("ViRef"=w966, "VIsToSerachFor/ViName"=w969, "error in (no error)"=w968) -> ("VisFound"=w973:refnum<vi>[], "error out"=w972:errorcluster)  [unwired: 15 in]
            n428 = Index Array(array=w973) -> (element=w975:refnum<vi>)  [unwired: 1 in]
            n429 = invoke class="GObj" method="Replace"(reference=w975, error in=w972, "Path"=w959) -> (error out=w976:errorcluster, "Replace"=w974:refnum<vi>)  [unwired: 3 in, 4 out]
            n430 = Close Reference(reference=w973, error in (no error)=w976) -> ()  [unwired: 1 out]
            n431 = Close Reference(reference=w974, error in (no error)=w976) -> (error out=w971:errorcluster)
            n432 = invoke class="VI" method="Save.Instrument"(reference=w966, error in=w971) -> (error out=w978:errorcluster)  [unwired: 4 in, 5 out]
          }
        }
        n433 = Equal?(x=w902, y="Exit") -> (x = y?=w905:bool)
        n434 = Select(t="Error", s=w901, f=w902) -> (s? t:f=w906:string)
      }
    }
  }
  "error out" <- w8
  "DataOut" <- w5
  "Cancelled" <- w6
  "Name" <- w1
